vi "Choix des parametres.vi"() -> ()   [LabVIEW 2022 SP3]
uses:
  Enum/Enum 3.ctl
  Variables globales/Variable glob mails.vi
  Variables globales/Variable glob generale.vi
  Variables globales/Variable glob Leybold.vi
  Variables globales/Variable glob Edwards.vi
  Variables globales/Variable glob Keller.vi
  Variables globales/Variable glob Th.vi
  Variables globales/Variable glob Pt.vi
  Variables globales/Variables glob EUROTHERM.vi
  Variables globales/Variable globale compteurs.vi
  <vilib>/Utility/config.llb/NI_LVConfig.lvlib
panel:
  out "CUVE":string
  out "Refnum VI":refnum<vi>
  out "sortie d'erreur":errorcluster
  in  "Commande onglets 2":T1(tab)=enum."Temperatures Th"
  in  "Mails autres":string[](array[string]) caption="Mails autres (a renseigner) :"
  in  "Adresses mail IAS :":i32[](listbox)=[5] caption="Adresses mail IAS pour alertes :\n(selection par double clic)"
  in  "Commentaire dans le fichier :":string caption="Écrire éventuellement un commentaire qui sera inséré dans l'entête du fichier :"
  in  "Sous-dossier eventuel":string caption="Nom de l'expérience"
  in  "Nom manip":string caption="Nom de l'experience"
  in  "Sous-dossier precedents":u16(ring) items=["", "TEST_VADER_AVRIL2018"]
  in  "Experiences precedentes":u16(ring) items=["arretdu140716", "CAMERA FSI FM", "CAMERA FSI QM", "CAMERA HRI EUV FM", "CAMERA HRI EUV FM 2", "CAMERA HRI Lya FM", "essai blancdu070316", "FiltreFSI4et26du180716", "FiltreFSIFMmiroir3du50916", "FiltreFSIFmn6du010816", "FiltreFSIn30du270716", "FiltreFSIn32du210716", "FiltreFSIn5du250716", "FiltreFSIn6du290716", "FSI140416", "FSI150416", "FSIfiltreFMn13et25", "FSIfiltreFMn26", "FSIfiltreFMn4et26", "FSIfiltreQM180516", "HRIdu141015", "HRIdu151015", "HRIdu191015", "HRIdu271015", "Miroir2FSIdu30516", "NeptnXR90i", "NeptnXR90itest2", "POMPE RECEPTION", "PompNeptnxr40i", "PrepaNeptEUI", "Profils de température", "RGA", "test ablanc", "Test cDAQ", "Test programme", "TEST_VADER", "Testblanccam1et2du031215", "testmontage a blanc camdu270916", "tests camdu270916", "TESTS_LS340", "testsablanc", "testsBlancdu290916", "Testscam1et2du110216", "Testscam1et2du1mars16", "Testscam1et2du21mars16", "testscam1et2du300316", "testscamdu040416", "Testscaméra080216", "Testscaméra290116", "testscrycooleretbrides", "TestsEchandu281116", "échantHriFsi031016"]
  out "Chemin DATA local":path caption="Chemin DATA local :"
  in  "Chemin DATA distant":path caption="Chemin DATA distant :"
  in  "Chemin sauvegarde":path caption="Chemin sauvegarde :"
  out "Ports COM LEYBOLD":refnum<visa-resource-name>[](array[refnum])
  in  "Nom des jauges\nLEYBOLD":string[](array[string])
  in  "Selection\nLEYBOLD":bool[](array[boolean])
  out "Val LEYBOLD":string[](array[string]) caption="Valeurs\nLEYBOLD\ninstantanees"
  out "Val Grappes":string[](array[string]) caption="Valeurs Grappes\ninstantanees"
  in  "Selection\nGrappes":bool[](array[boolean])
  in  "Grappes":string[][](array[string])
  out "Ports COM EDWARDS":refnum<visa-resource-name>[](array[refnum])
  in  "Selection EDWARDS":bool[][](array[boolean])
  in  "Nom des jauges EDWARDS":string[][](array[string])
  out "Val EDWARDS":string[][](array[string]) caption="Valeurs EDWARDS instantanees"
  out "Nom de la tache Th associee":refnum<k21>
  in  "Tableau Th":T2(array[cluster])=[{"Test Th"=[], "Selection Th"=[TRUE, TRUE, FALSE, FALSE, TRUE, TRUE, FALSE, FALSE], "Tableau"=["Th1", "Th2", "Th3", "Th4", "Th5", "Th6", "Th7", "Th8"], "Noms Thermocouples :"=["SCXI1-Th1", "SCXI1-Th2", "SCXI1-Th3", "SCXI1-Th4", "SCXI1-Th5", "SCXI1-Th6", "SCXI1-Th7", "SCXI1-Th8"]}, {"Test Th"=[], "Selection Th"=[TRUE, TRUE, TRUE, TRUE, TRUE, TRUE, TRUE, TRUE], "Tableau"=["Th1", "Th2", "Th3", "Th4", "Th5", "Th6", "Th7", "Th8"], "Noms Thermocouples :"=["Thermocouple1", "Thermocouple2", "Thermocouple3", "Thermocouple4", "Thermocouple5", "Thermocouple6", "Thermocouple7", "Thermocouple8"]}]
  in  "Th n°":u8=1 caption="chassis n°" min=1
  in  "Tableau Pt":T3(array[cluster])=[{"Test Pt"=[], "Sélection Pt"=[TRUE, TRUE, FALSE, FALSE, TRUE, TRUE, FALSE, FALSE], "Tableau"=["Th1", "Th2", "Th3", "Th4", "Th5", "Th6", "Th7", "Th8"], "Noms Platines :"=["SCXI1-Th1", "SCXI1-Th2", "SCXI1-Th3", "SCXI1-Th4", "SCXI1-Th5", "SCXI1-Th6", "SCXI1-Th7", "SCXI1-Th8"]}, {"Test Pt"=[], "Sélection Pt"=[TRUE, TRUE, TRUE, TRUE, TRUE, TRUE, TRUE, TRUE], "Tableau"=["Th1", "Th2", "Th3", "Th4", "Th5", "Th6", "Th7", "Th8"], "Noms Platines :"=["Thermocouple1", "Thermocouple2", "Thermocouple3", "Thermocouple4", "Thermocouple5", "Thermocouple6", "Thermocouple7", "Thermocouple8"]}]
  in  "Pt n°":u8=1 caption="chassis n°" min=1
  out "Nom de la tache Pt associee":refnum<k21>
  out "Donnees reg":T4(array[cluster])
  in  "Reg dispo":T5(array[cluster])
  in  "Port COM REG":u16(ring) items=["COM6"]
  out "Adresses des jauges":i16[](array[numeric])
  out "Port COM KELLER (RS485)":refnum<visa-resource-name>
  out "Val KELLER":string[](array[string]) caption="Valeurs\nKELLER\ninstantanees"
  in  "Selection\nKELLER":bool[](array[boolean])
  in  "Nom des jauges KELLER":string[](array[string])
  in  "Temps pour débit":u16=3601 caption="Intervale de temps (s) pour debit" min=1
  out "data compteurs":string[](array[string])
  in  "Init compteurs (m3)":dbl[](array[numeric]) format="%.2f"
  in  "Selection":bool[](array[boolean])
  out "Noms des compteurs":string[](array[string])
  out "Nom de la tâche compteurs":refnum<k21>
  in  "annuler":bool
  in  "stop":bool
  # "choix des parametres"
  # "Ce logiciel et les informations qu'il contient, sont la propriété de l’IAS et ne peuvent être diffusés sans l’autorisation de la Station d’étalonnage"
  # "LES VALEURS AFFICHEES DANS LES TABLEAUX \"TEST\" CORRESPONDENT A UNE ACQUISITION TOUTES LES\nSECONDES SANS ENREGISTREMENT\n\nSEULES LES VOIES SÉLECTIONNEES SERONT ENSUITE ENREGISTREES"
  # "Définition du nom du dossier d'enregistrement des données.\nChoisir dans la liste de gauche ou écrire un nouveau nom dans la case de droite.\n\nLes fichiers seront écrits dans : D:\\Data\\CUVE\\Expérience\\(Sous-dossier\\)Année\\mois"
  # "Sélectionner les thermocouples"
  # "Sélectionner les platines du cDAQ"
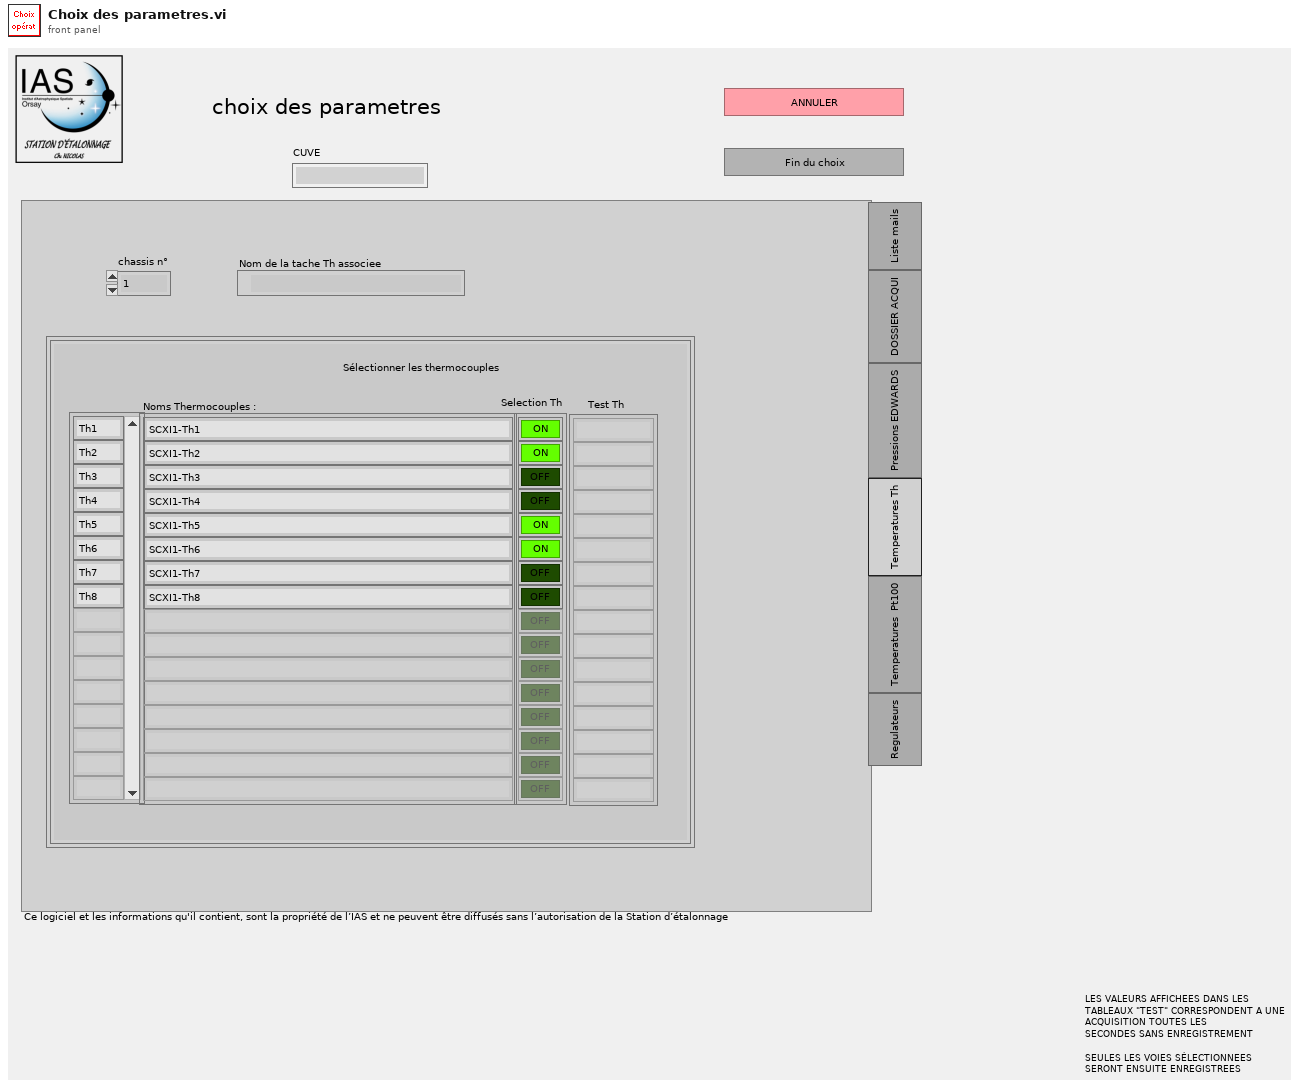
[diagram p1: front panel]
types:
  T1 = enum32{"Liste mails", "DOSSIER ACQUI", "Pressions LEYBOLD", "Pressions EDWARDS", "Temperatures Th", "Temperatures  Pt100", "Regulateurs", "Pressions KELLER", "Compteurs"}
  T2 = cluster{"Test Th":string[], "Selection Th":bool[], "Tableau":string[], "Noms Thermocouples :":string[]}[]
  T3 = cluster{"Test Pt":string[], "Sélection Pt":bool[], "Tableau":string[], "Noms Platines :":string[]}[]
  T4 = cluster{"Données  1 COM":cluster{"Pt100 Mesure":string, "Pt100 Securite":string}[]}[]
  T5 = cluster{"1 COM reg":cluster{"Nom":string, "Adresse":u8, "sélect":bool}[]}[]
  T6 = typedef "Enum 3.ctl" = enum16{"init", "init mail", "acquisition en cours ?", "onglets visibles", "init pressions", "initTh", "init Pt", "init reg", "init compteurs", "init dossiers", "lancement acqui tout", "choix operateur", "arret acquisitions", "enregistrement var glob pres", "enregistrement var glob temp", "enregistrement var glob reg", "enregistrement var glob compt et dossiers", "creation dossiers", "enregistrement fichier config", "fin"}
  T7 = cluster{"Données  1 COM":cluster{"Pt100 Mesure":string, "Pt100 Sécurité":string}[]}[]
  T8 = cluster{"Nom":string, "Adresse":u8, "sélect":bool}[]
  T9 = cluster{"Pt Mesure":string, "Pt Sécurité":string}
  T10 = enum32{"Invalid", "Standard", "Closed", "Hidden", "Minimized", "Maximized"}
  T11 = typedef "LVPositionTypeDef.ctl" = cluster{"Left":i32, "Top":i32}
  T12 = typedef "LVBoundsTypeDef.ctl" = cluster{"Width":u32, "Height":u32}
  T13 = cluster{"Nom tache Th":refnum<k21>, "Noms des Th":string[], "Nb Th":i16, "Selection Th":bool[], "Nom Th selectionnes":string[]}[]
  T14 = cluster{"Test Th":string[], "Selection Th":bool[], "Tableau":string[], "Noms Thermocouples :":string[]}
  T15 = cluster{"Nom tache Pt":refnum<k21>, "Noms des Pt":string[], "Nb Pt":i16, "Selection Pt":bool[], "Nom Pt selectionnees":string[]}[]
  T16 = cluster{"Test Pt":string[], "Sélection Pt":bool[], "Tableau":string[], "Noms Platines :":string[]}
  T17 = cluster{"1 COM reg":cluster{"Nom":string, "Adresse":u8, "sélect":bool}[]}
  T18 = cluster{"Nom":string, "Adresse":u8, "sélect":bool}
  T19 = cluster{"Nom tache compteurs":refnum<k21>, "Noms des compteurs":string[], "Selection":bool[], "Init compteurs":dbl[], "Noms compteurs selectionnes":string[]}
  T20 = cluster{cluster{"Pt Mesure":string, "Pt Sécurité":string}[]}
  T21 = cluster{"Nom tache Th":refnum<k21>, "Noms des Th":string[], "Nb Th":i16, "Selection Th":bool[], "Nom Th selectionnes":string[]}
  T22 = cluster{"Nom tache Pt":refnum<k21>, "Noms des Pt":string[], "Nb Pt":i16, "Selection Pt":bool[], "Nom Pt selectionnees":string[]}
  T23 = typedef "NI_LVConfig.lvlib/Config Data RefNum.ctl" = refnum<k1>
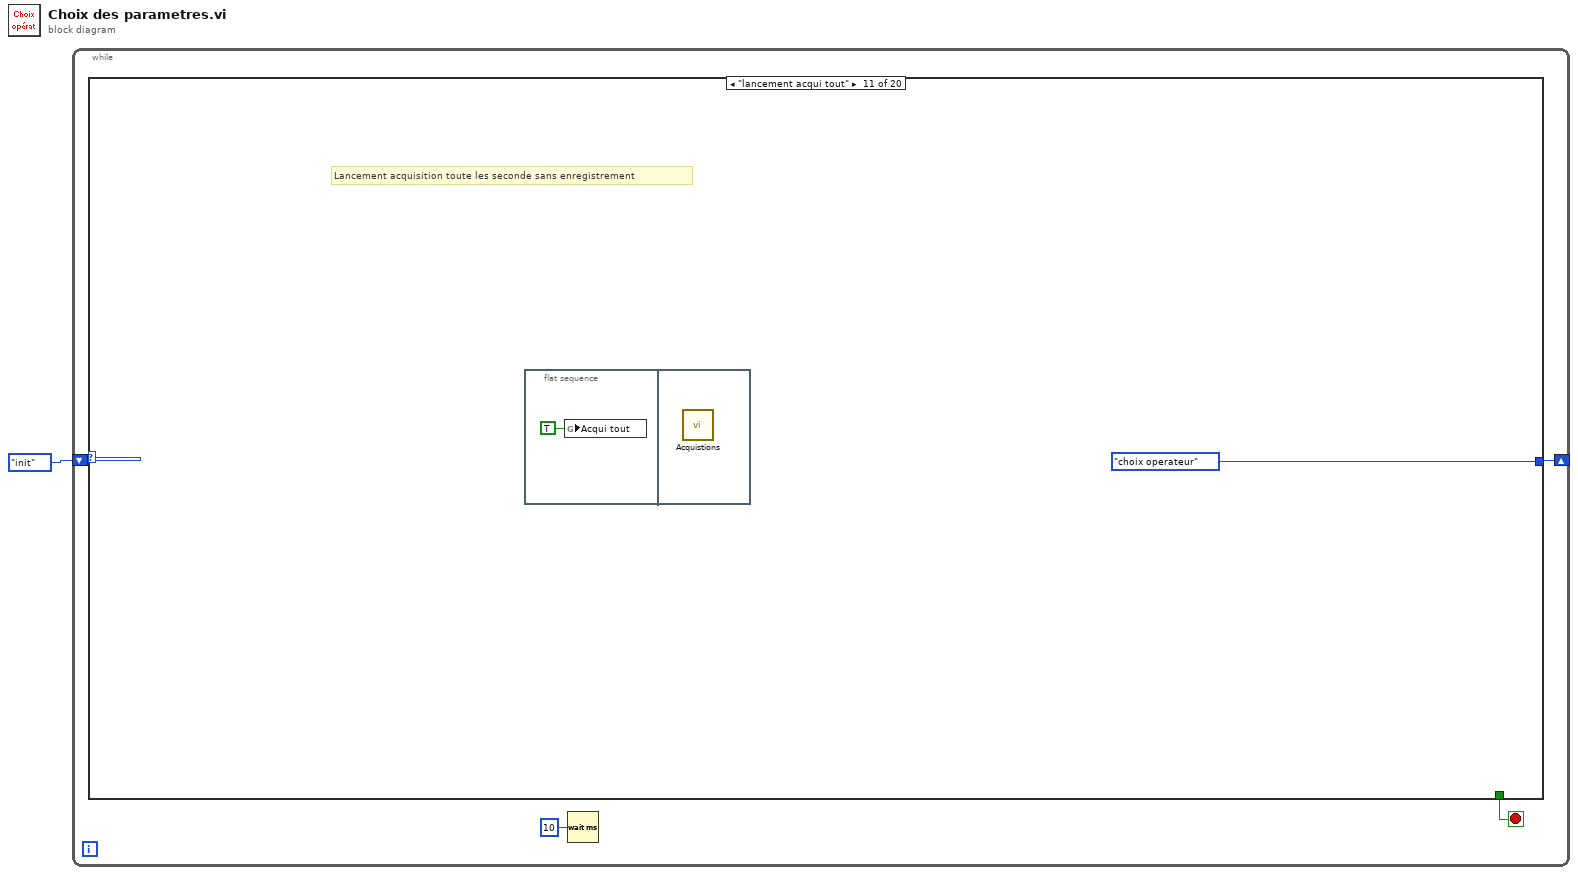
[diagram p0: block diagram]
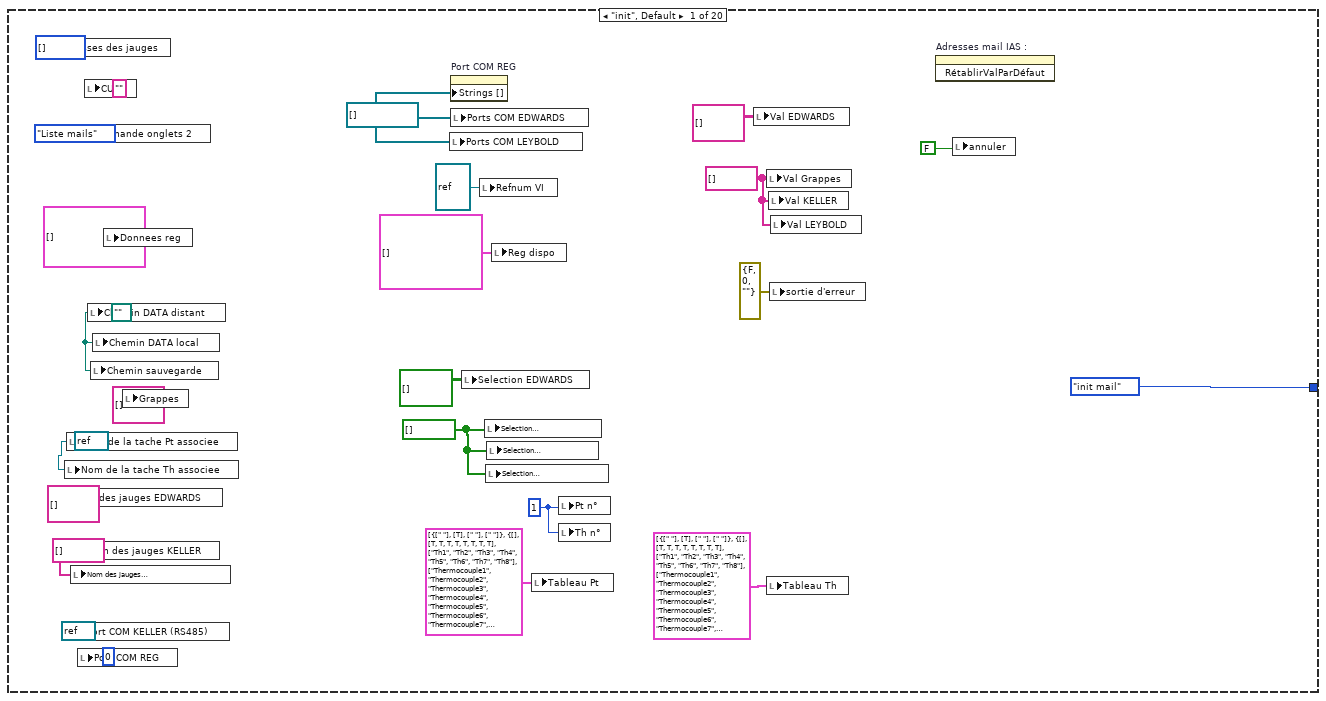
[diagram p2: hidden frame]
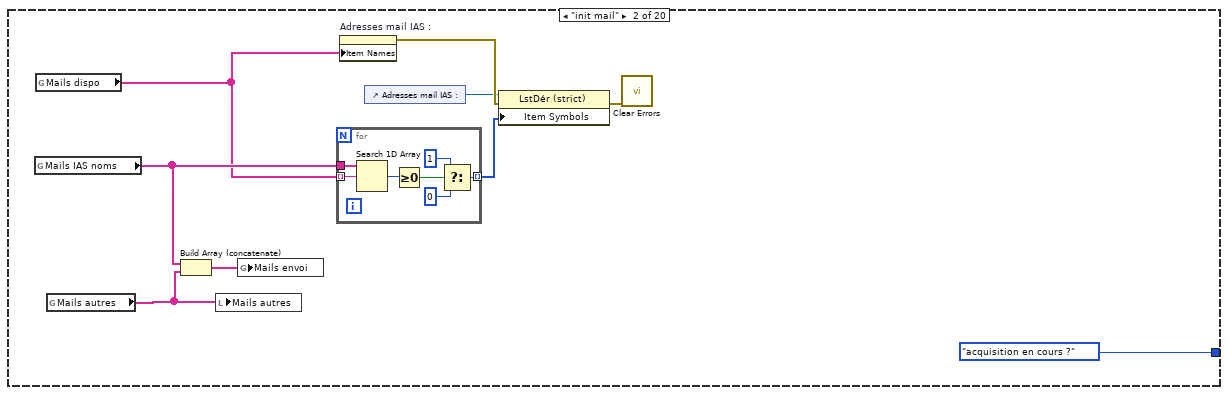
[diagram p3: hidden frame]
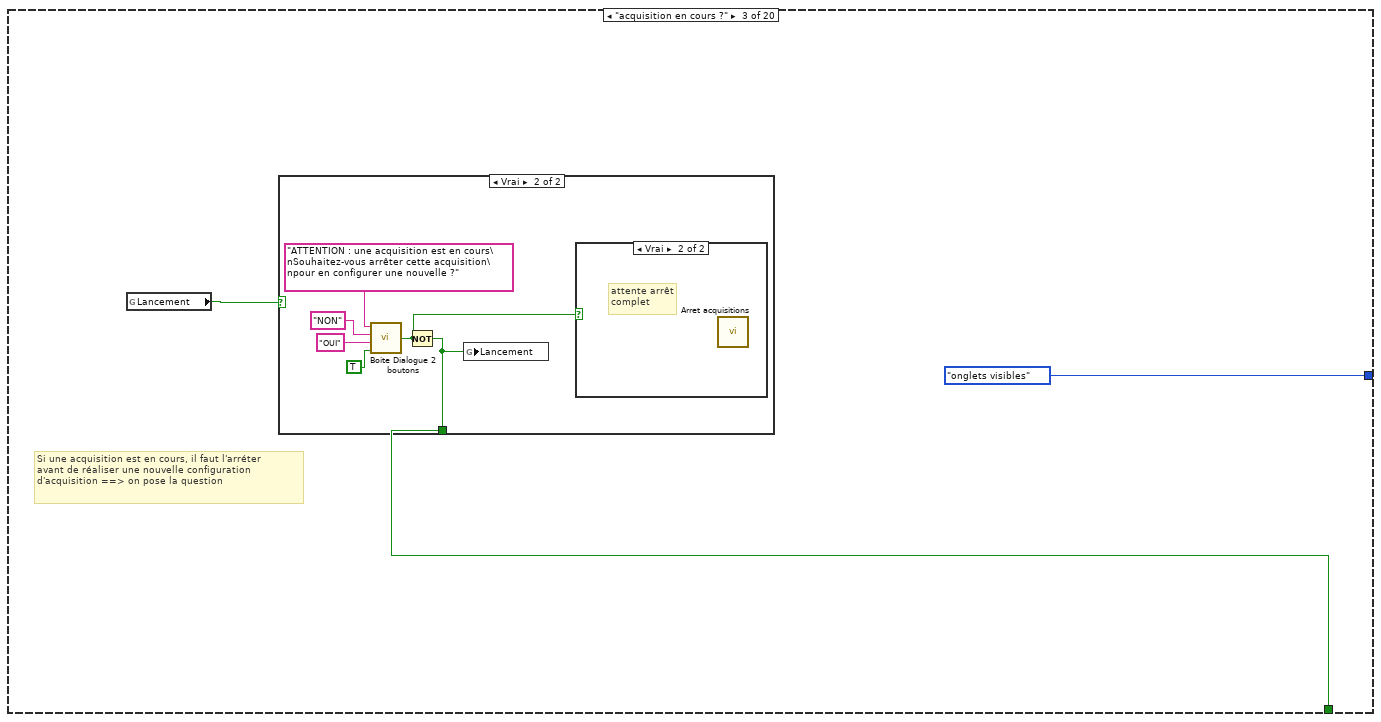
[diagram p4: hidden frame]
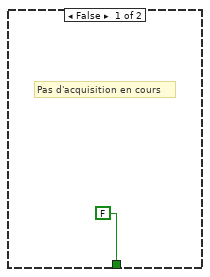
[diagram p5: hidden frame]
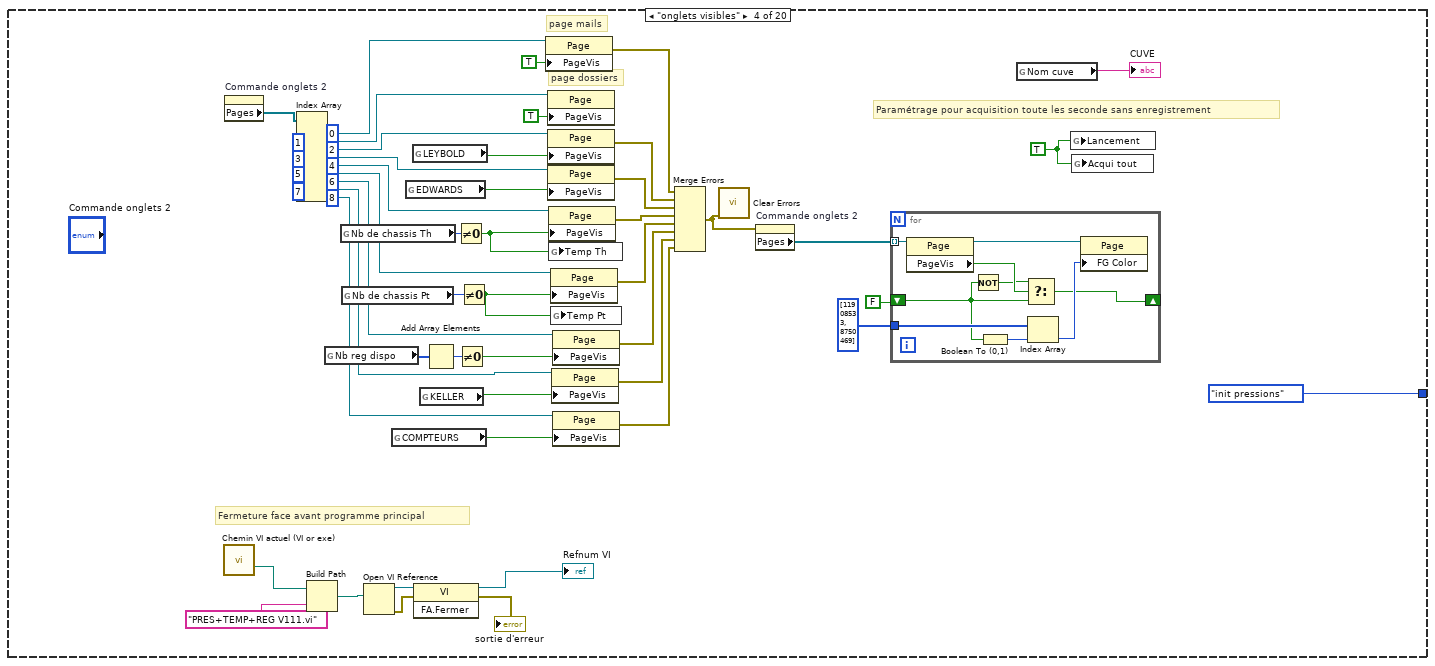
[diagram p7: hidden frame]
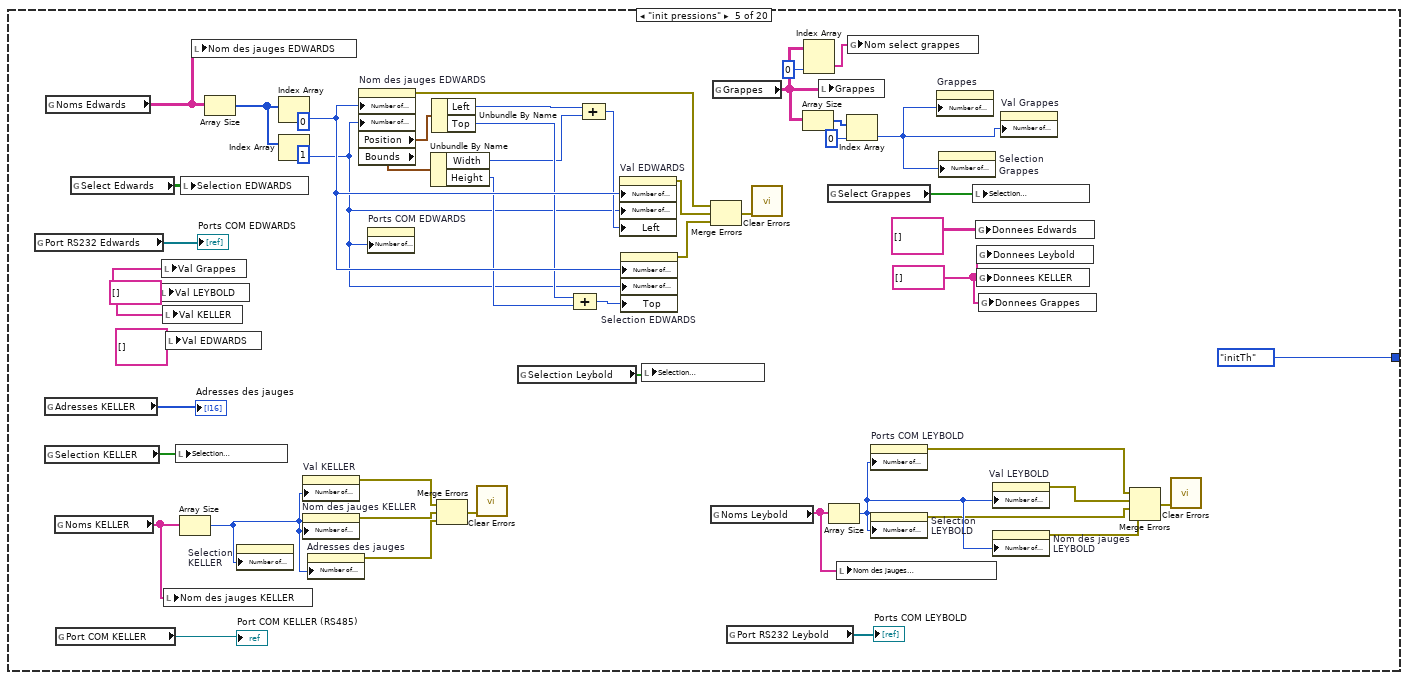
[diagram p8: hidden frame]
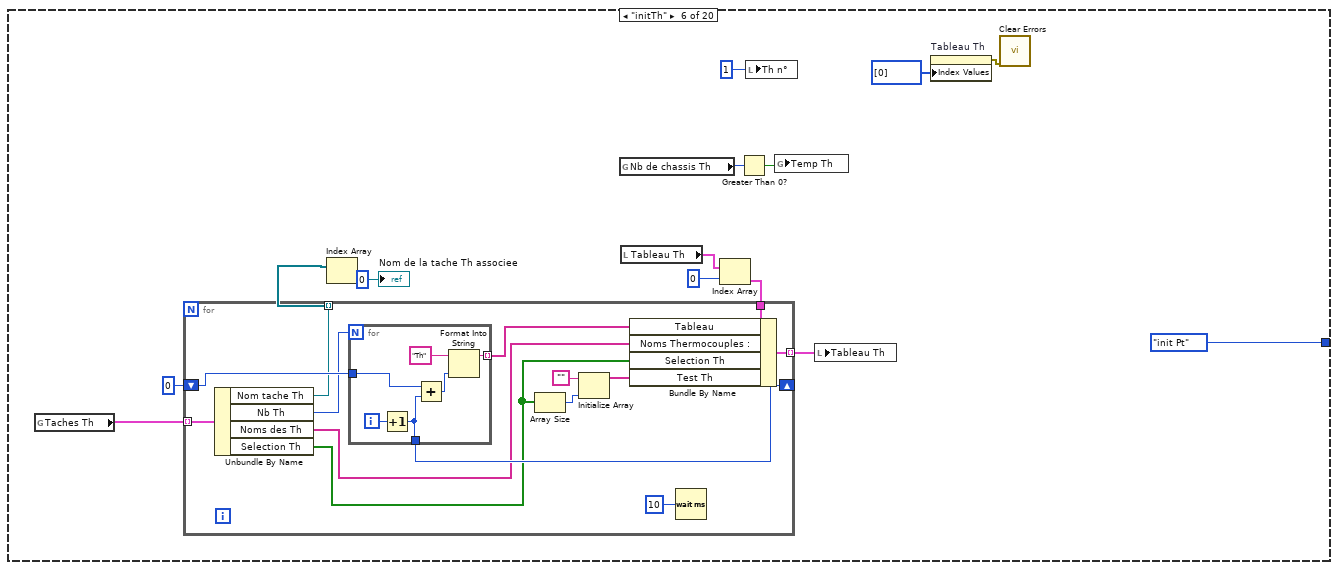
[diagram p9: hidden frame]
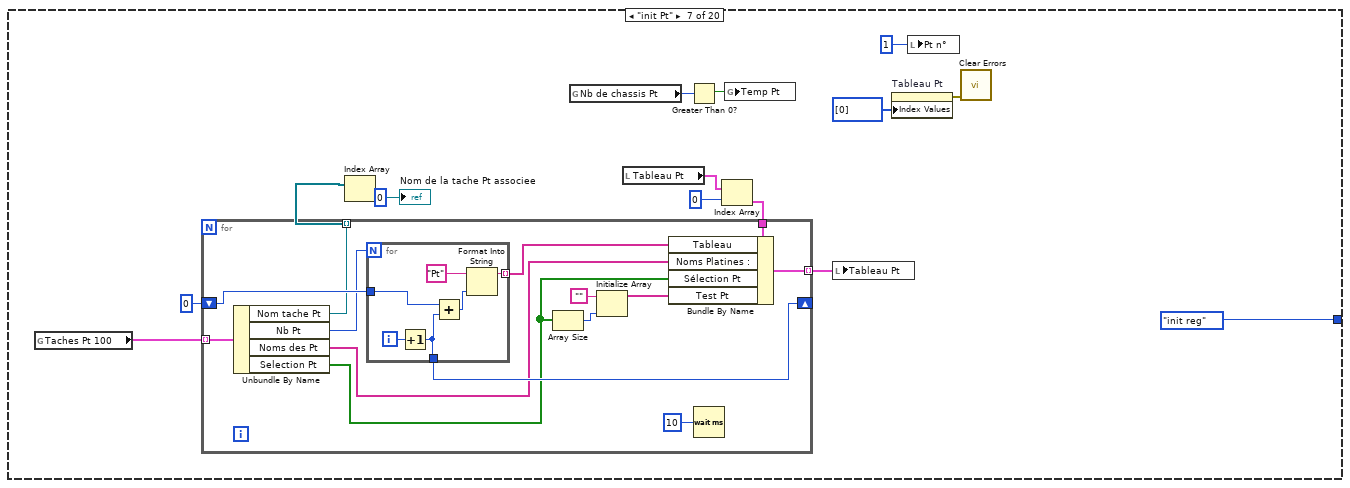
[diagram p10: hidden frame]
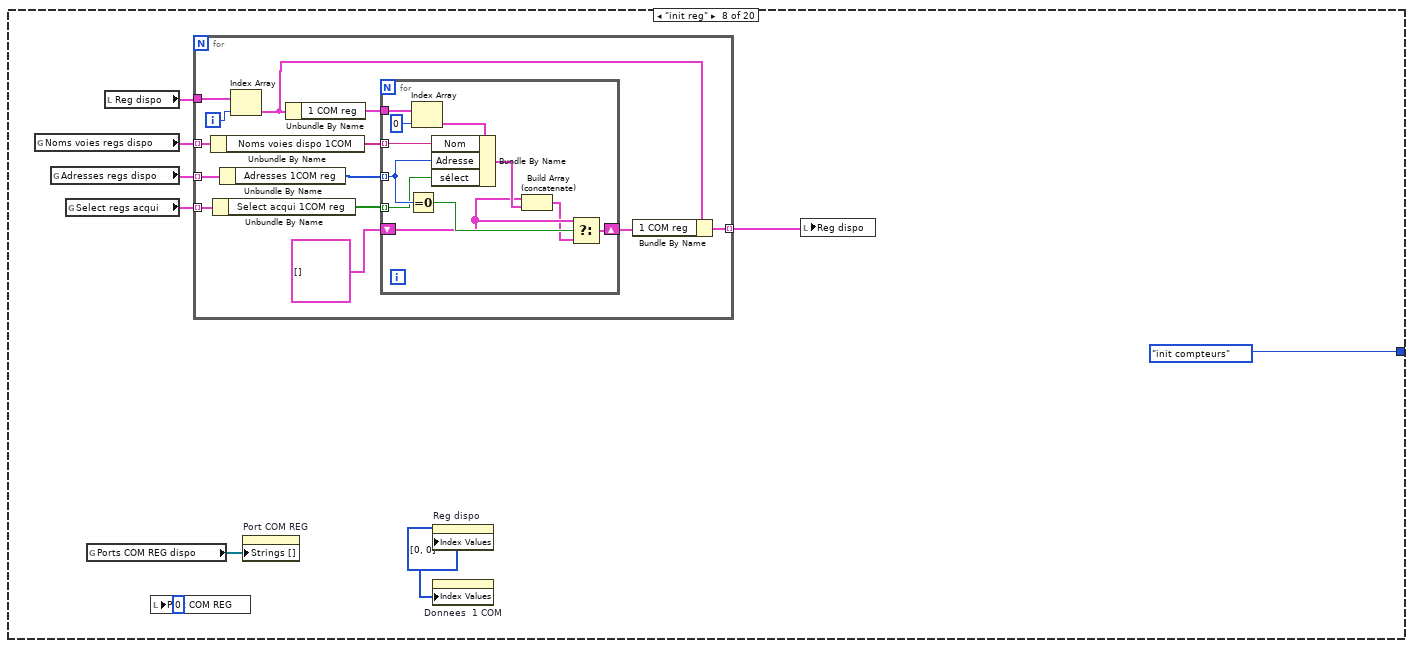
[diagram p11: hidden frame]
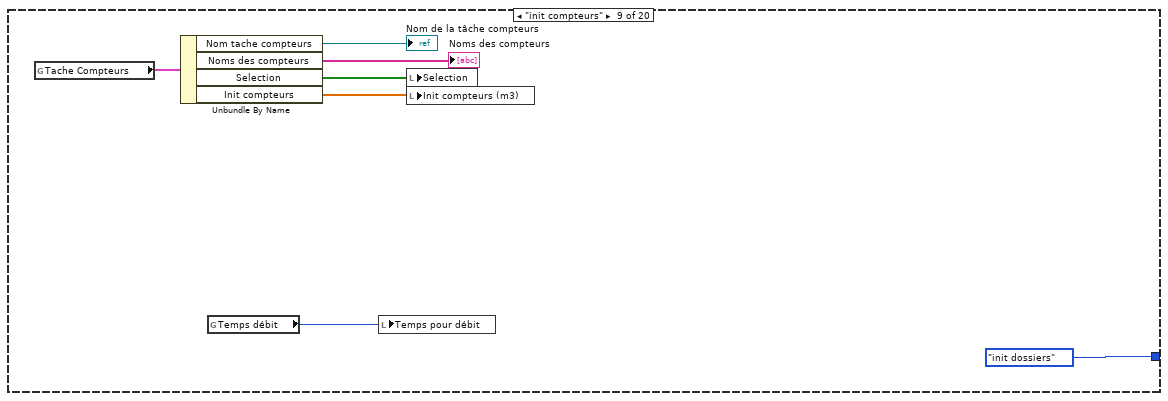
[diagram p12: hidden frame]
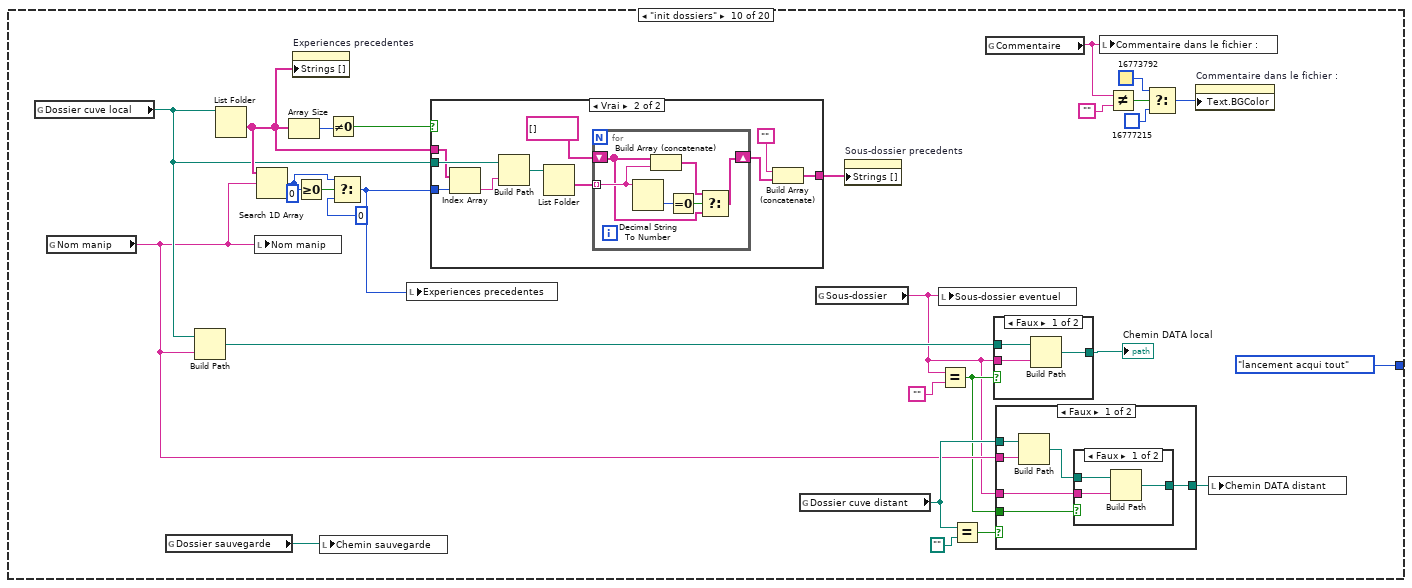
[diagram p13: hidden frame]
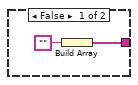
[diagram p17: hidden frame]
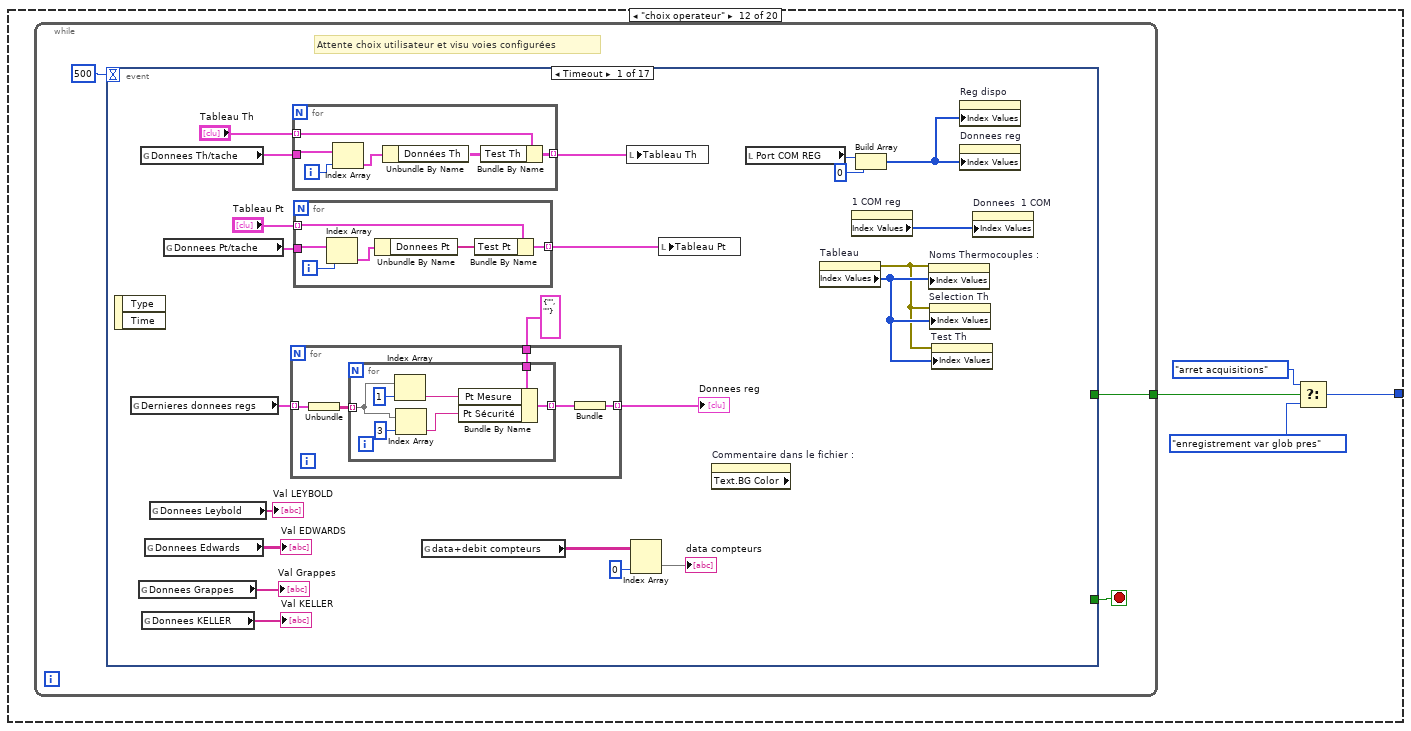
[diagram p18: hidden frame]
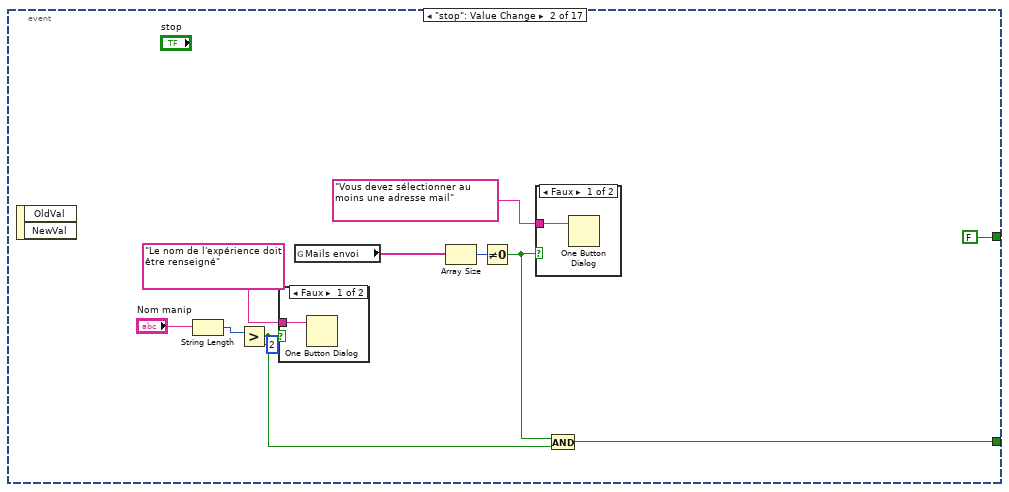
[diagram p19: hidden frame]
diagram:
  n1 = while {
    shift-right: [w4] -> _
    shift-left: Enum_3."init" ("Énum") -> [w5]
    stop <- w3 stop-if-true
    n2 = case shown="\"lancement acqui tout\"" w5 {
      tunnel: [Enum_3."init mail" ("Énum") Enum_3."acquisition en cours ?" ("Énum") Enum_3."onglets visibles" ("Énum") Enum_3."init pressions" ("Énum") Enum_3."initTh" ("Énum") Enum_3."init Pt" ("Énum") Enum_3."init reg" ("Énum") Enum_3."init compteurs" ("Énum") Enum_3."init dossiers" ("Énum") Enum_3."lancement acqui tout" ("Énum") Enum_3."choix operateur" ("Énum") w342 Enum_3."enregistrement var glob temp" ("Énum") Enum_3."enregistrement var glob reg" ("Énum") Enum_3."enregistrement var glob compt et dossiers" ("Énum") Enum_3."creation dossiers" ("Énum") Enum_3."enregistrement fichier config" ("Énum") Enum_3."arret acquisitions" ("Énum") Enum_3."fin" ("Énum") Enum_3."acquisition en cours ?" ("Énum")] -> w4
      tunnel: [_ _ w47 _ _ _ _ _ _ _ _ _ _ _ _ _ _ _ _ TRUE] -> w3
      frame "init", Default {
        w16 = string[] [] ("Val Grappes")
        w19 = bool[] [] ("Sélection\nGrappes")
        w10 = refnum<visa-resource-name>[] [] ("Ports COM EDWARDS")
        w23 = string[] [] ("Nom des jauges KELLER")
        w22 = refnum<k21> refnum ("Nom de la tâche Pt associée")
        w26 = path "" ("Dossier DATA distant")
        w18 = u8 1 ("Pt n°")
        n3 = local write "Adresses des jauges"(i16[] [] ("Adresses des jauges")) -> ()
        n4 = local write "Nom des jauges EDWARDS"(string[][] [] ("Nom des jauges EDWARDS")) -> ()
        n5 = local write "Nom de la tache Th associee"(w22) -> ()
        n6 = local write "Nom de la tache Pt associee"(w22) -> ()
        n7 = local write "Nom des jauges KELLER"(w23) -> ()
        n8 = local write "Nom des jauges\nLEYBOLD"(w23) -> ()
        n9 = local write "Port COM KELLER (RS485)"(refnum<visa-resource-name> refnum ("Port COM JUMO (RS485)")) -> ()
        n10 = local write "Commande onglets 2"(T1."Liste mails" ("Commande onglets 2")) -> ()
        n11 = local write "Port COM REG"(u16 0) -> ()
        n12 = local write "CUVE"("" ("CUVE")) -> ()
        n13 = local write "Chemin DATA distant"(w26) -> ()
        n14 = local write "Chemin sauvegarde"(w26) -> ()
        n15 = local write "Chemin DATA local"(w26) -> ()
        n16 = local write "Donnees reg"(T7 [] ("Donnees reg")) -> ()
        n17 = local write "Grappes"(string[][] [] ("Grappes")) -> ()
        n18 = local write "Ports COM LEYBOLD"(w10) -> ()
        n19 = property on="Port COM REG" class="MDér (strict)"("Strings []"=w10) -> ()  [unwired: 2 in, 2 out]
        n20 = local write "Ports COM EDWARDS"(w10) -> ()
        n21 = local write "Selection EDWARDS"(bool[][] [] ("Sélection EDWARDS")) -> ()
        n22 = local write "Refnum VI"(refnum<vi> refnum ("Refnum VI")) -> ()
        n23 = local write "Selection\nGrappes"(w19) -> ()
        n24 = local write "Selection\nLEYBOLD"(w19) -> ()
        n25 = local write "Selection\nKELLER"(w19) -> ()
        n26 = local write "Reg dispo"(T5 [] ("Reg dispo")) -> ()
        n27 = local write "Tableau Pt"(T3 [{"Test Pt"=[" "], "Sélection Pt"=[TRUE], "Tableau"=[" "], "Noms Platines :"=[" "]}, {"Test Pt"=[], "Sélection Pt"=[TRUE, TRUE, TRUE, TRUE, TRUE, TRUE, TRUE, TRUE], "Tableau"=["Th1", "Th2", "Th3", "Th4", "Th5", "Th6", "Th7", "Th8"], "Noms Platines :"=["Thermocouple1", "Thermocouple2", "Thermocouple3", "Thermocouple4", "Thermocouple5", "Thermocouple6", "Thermocouple7", "Thermocouple8"]}] ("Tableau Pt")) -> ()
        n28 = local write "Pt n°"(w18) -> ()
        n29 = local write "Th n°"(w18) -> ()
        n30 = local write "Val EDWARDS"(string[][] [] ("Val EDWARDS")) -> ()
        n31 = local write "Val Grappes"(w16) -> ()
        n32 = local write "Tableau Th"(T3 [{"Test Pt"=[" "], "Sélection Pt"=[TRUE], "Tableau"=[" "], "Noms Platines :"=[" "]}, {"Test Pt"=[], "Sélection Pt"=[TRUE, TRUE, TRUE, TRUE, TRUE, TRUE, TRUE, TRUE], "Tableau"=["Th1", "Th2", "Th3", "Th4", "Th5", "Th6", "Th7", "Th8"], "Noms Platines :"=["Thermocouple1", "Thermocouple2", "Thermocouple3", "Thermocouple4", "Thermocouple5", "Thermocouple6", "Thermocouple7", "Thermocouple8"]}] ("Tableau Pt")) -> ()
        n33 = local write "Val KELLER"(w16) -> ()
        n34 = local write "sortie d'erreur"(errorcluster {"status"=FALSE, "code"=0, "source"=""} ("sortie d'erreur")) -> ()
        n35 = local write "Val LEYBOLD"(w16) -> ()
        n36 = invoke on="Adresses mail IAS :" class="LstDér (strict)" method="RétablirValParDéfaut"() -> ()  [unwired: 3 in, 3 out]
        n37 = local write "annuler"(FALSE) -> ()
      }
      frame "init mail" {
        n38 = global read "Variable glob mails.vi" "Mails IAS noms"() -> (w33:string[])
        n39 = global read "Variable glob mails.vi" "Mails dispo"() -> (w30:string[])
        n40 = global read "Variable glob mails.vi" "Mails autres"() -> (w32:string[])
        n41 = Build Array (concatenate)(w33, w32) -> (w31:string[])
        n42 = local write "Mails autres"(w32) -> ()
        n43 = global write "Variable glob mails.vi" "Mails envoi"(w31) -> ()
        n44 = for {
          tunnel: w33 -> [w45]
          tunnel: w30 -> [w44] mode=indexing
          tunnel: [w39] -> w35 mode=indexing
          n45 = Search 1D Array(1D array=w45, element=w44) -> (index of element=w43:i32)  [unwired: 1 in]
          n46 = Greater Or Equal To 0?(x=w43) -> (x >= 0?=w42:bool)
          n47 = Select(t=1 ("cas vrai"), s=w42, f=0) -> (s? t:f=w39:i32)
        }
        n48 = property on="Adresses mail IAS :" class="LstDér (strict)"("Item Names"=w30) -> (error out=w36:errorcluster)  [unwired: 2 in, 1 out]
        n49 = control-ref of="Adresses mail IAS :"() -> (w34:refnum<vi>)
        n50 = property class="LstDér (strict)"(reference=w34, error in=w36, "Item Symbols"=w35) -> (error out=w37:errorcluster)  [unwired: 1 out]
        n51 = call <vilib>:"Clear Errors.vi"("error in (no error)"=w37) -> ()  [unwired: 5 in, 2 out]
      }
      frame "acquisition en cours ?" {
        # "Si une acquisition est en cours, il faut l'arréter\navant de réaliser une nouvelle configuration\nd'acquisition ==> on pose la question"
        n52 = global read "Variable glob generale.vi" "Lancement"() -> (w48:bool)
        n53 = case shown="Vrai" w48 {
          tunnel: [FALSE w55] -> w47
          frame False {
            # "Pas d'acquisition en cours"
          }
          frame True {
            n54 = call "Boite Dialogue 2 boutons.vi"("bouton droit visible ?"=TRUE, "Texte bouton droit"="OUI" ("Nom du bouton V (\"OK\")"), "Texte bouton gauche"="NON" ("Nom du bouton F (\"Annuler\")"), "Message"="ATTENTION : une acquisition est en cours\nSouhaitez-vous arrêter cette acquisition\npour en configurer une nouvelle ?" ("message")) -> ("Bouton droit ?"=w51:bool)
            n55 = Not(x=w51) -> (.not. x?=w55:bool)
            n56 = global write "Variable glob generale.vi" "Lancement"(w55) -> ()
            n57 = case shown="Vrai" w51 {
              frame False {
              }
              frame True {
                # "attente arrêt\ncomplet"
                n58 = call "Arret acquisitions.vi"() -> ()  [unwired: 12 in]
              }
            }
          }
        }
      }
      frame "onglets visibles" {
        w99 = TRUE
        # "page dossiers"
        # "page mails"
        # "Paramétrage pour acquisition toute les seconde sans enregistrement"
        # "Fermeture face avant programme principal"
        n59 = call "Chemin VI actuel (VI or exe).vi"() -> ("VI or executable installation directory"=w83:path)  [unwired: 14 in, 1 out]
        n60 = property on="Commande onglets 2" class="Onglet (strict)"() -> ("Pages"=w109:refnum<vi>[])  [unwired: 2 in, 2 out]
        n61 = Index Array(array=w109, index #1=0 ("indice"), index #2=1 ("indice"), index #3=2 ("indice"), index #4=3 ("indice"), index #5=4 ("indice"), index #6=5 ("indice"), index #7=6 ("indice"), index #8=7 ("indice"), index #9=8 ("indice")) -> (element #1=w79:refnum<vi>, element #2=w64:refnum<vi>, element #3=w63:refnum<vi>, element #4=w62:refnum<vi>, element #5=w61:refnum<vi>, element #6=w60:refnum<vi>, element #7=w59:refnum<vi>, element #8=w58:refnum<vi>, element #9=w56:refnum<vi>)
        n62 = Build Path(base path=w83, name or relative path="PRES+TEMP+REG V111.vi" ("nom ou chemin relatif")) -> (appended path=w95:path)
        n63 = global read "Variables glob EUROTHERM.vi" "Nb reg dispo"() -> (w81:u8[])
        n64 = global read "Variable glob Th.vi" "Nb de chassis Th"() -> (w107:u8)
        n65 = global read "Variable glob Pt.vi" "Nb de chassis Pt"() -> (w108:u8)
        n66 = Open VI Reference(vi path=w95) -> (vi reference=w93:refnum<vi>, error out=w92:errorcluster)  [unwired: 5 in]
        n67 = global read "Variable globale compteurs.vi" "COMPTEURS"() -> (w71:bool)
        n68 = global read "Variable glob Edwards.vi" "EDWARDS"() -> (w106:bool)
        n69 = global read "Variable glob Leybold.vi" "LEYBOLD"() -> (w105:bool)
        n70 = invoke class="VI" method="FA.Fermer"(reference=w93, error in=w92) -> (reference out=→"Refnum VI":refnum<vi>, error out=→"sortie d'erreur":errorcluster)  [unwired: 1 in, 1 out]
        n71 = global read "Variable glob Keller.vi" "KELLER"() -> (w66:bool)
        n72 = Add Array Elements(numeric array=w81) -> (sum=w80:u8)
        n73 = Not Equal To 0?(x=w107) -> (x != 0?=w69:bool)
        n74 = Not Equal To 0?(x=w80) -> (x != 0?=w67:bool)
        n75 = Not Equal To 0?(x=w108) -> (x != 0?=w68:bool)
        n76 = property class="Page"(reference=w79, "PageVis"=TRUE ("Page visible")) -> (error out=w77:errorcluster)  [unwired: 1 in, 1 out]
        n77 = property class="Page"(reference=w64, "PageVis"=TRUE ("Page visible")) -> ()  [unwired: 1 in, 2 out]
        n78 = property class="Page"(reference=w63, "PageVis"=w105) -> (error out=w91:errorcluster)  [unwired: 1 in, 1 out]
        n79 = property class="Page"(reference=w62, "PageVis"=w106) -> (error out=w88:errorcluster)  [unwired: 1 in, 1 out]
        n80 = property class="Page"(reference=w61, "PageVis"=w69) -> (error out=w87:errorcluster)  [unwired: 1 in, 1 out]
        n81 = global write "Variable glob Th.vi" "Temp Th"(w69) -> ()
        n82 = property class="Page"(reference=w60, "PageVis"=w68) -> (error out=w89:errorcluster)  [unwired: 1 in, 1 out]
        n83 = global write "Variable glob Pt.vi" "Temp Pt"(w68) -> ()
        n84 = property class="Page"(reference=w58, "PageVis"=w66) -> (error out=w84:errorcluster)  [unwired: 1 in, 1 out]
        n85 = property class="Page"(reference=w59, "PageVis"=w67) -> (error out=w90:errorcluster)  [unwired: 1 in, 1 out]
        n86 = property class="Page"(reference=w56, "PageVis"=w71) -> (error out=w70:errorcluster)  [unwired: 1 in, 1 out]
        n87 = Merge Errors(w77, w91, w88, w87, w89, w90, w84, w70) -> (w74:errorcluster)
        n88 = call <vilib>:"Clear Errors.vi"("error in (no error)"=w74) -> ()  [unwired: 5 in, 2 out]
        n89 = property on="Commande onglets 2" class="Onglet (strict)"(error in=w74) -> ("Pages"=w76:refnum<vi>[])  [unwired: 1 in, 2 out]
        n90 = for {
          tunnel: w76 -> [w118] mode=indexing
          tunnel: u32[] [11908533, 8750469] ("Tableau") -> [w115]
          shift-right: [w110] -> _
          shift-left: FALSE -> [w111]
          n91 = property class="Page"(reference=w118) -> (reference out=w117:refnum<vi>, "PageVis"=w116:bool)  [unwired: 1 in, 1 out]
          n92 = Not(x=w111) -> (.not. x?=w112:bool)
          n93 = Boolean To (0,1)(Boolean=w111) -> (0, 1=w113:i16)
          n94 = Select(t=w112, s=w116, f=w111) -> (s? t:f=w110:bool)
          n95 = Index Array(array=w115, index=w113) -> (element=w114:u32)
          n96 = property class="Page"(reference=w117, "FG Color"=w114) -> ()  [unwired: 1 in, 2 out]
        }
        n97 = global read "Variable glob generale.vi" "Nom cuve"() -> (→"CUVE":string)
        n98 = global write "Variable glob generale.vi" "Lancement"(w99) -> ()
        n99 = global write "Variable glob generale.vi" "Acqui tout"(w99) -> ()
      }
      frame "init pressions" {
        w125 = string[] [] ("Données KELLER")
        w126 = string[] [] ("Valeurs\nLEYBOLD\ninstantanées")
        n100 = global read "Variable glob Edwards.vi" "Port RS232 Edwards"() -> (→"Ports COM EDWARDS":refnum<visa-resource-name>[])
        n101 = global read "Variable glob Keller.vi" "Adresses KELLER"() -> (→"Adresses des jauges":i16[])
        n102 = global read "Variable glob Keller.vi" "Selection KELLER"() -> (w168:bool[])
        n103 = global read "Variable glob Edwards.vi" "Noms Edwards"() -> (w153:string[][])
        n104 = global read "Variable glob Keller.vi" "Noms KELLER"() -> (w152:string[])
        n105 = global read "Variable glob Keller.vi" "Port COM KELLER"() -> (→"Port COM KELLER (RS485)":refnum<visa-resource-name>)
        n106 = global read "Variable glob Edwards.vi" "Select Edwards"() -> (w166:bool[][])
        n107 = local write "Val LEYBOLD"(w126) -> ()
        n108 = local write "Val Grappes"(w126) -> ()
        n109 = local write "Val KELLER"(w126) -> ()
        n110 = local write "Nom des jauges KELLER"(w152) -> ()
        n111 = local write "Val EDWARDS"(string[][] [] ("Valeurs EDWARDS instantanées")) -> ()
        n112 = local write "Selection\nKELLER"(w168) -> ()
        n113 = Array Size(array=w152) -> (size(s)=w144:i32)
        n114 = local write "Selection EDWARDS"(w166) -> ()
        n115 = local write "Nom des jauges EDWARDS"(w153) -> ()
        n116 = Array Size(array=w153) -> (size(s)=w154:i32[])
        n117 = property on="Selection\nKELLER" class="Tabl (strict)"("Number of Rows"=w144) -> ()  [unwired: 2 in, 2 out]
        n118 = Index Array(array=w154, index=0 ("indice")) -> (element=w165:i32)
        n119 = Index Array(array=w154, index=1 ("indice")) -> (element=w147:i32)
        n120 = property on="Val KELLER" class="Tabl (strict)"("Number of Rows"=w144) -> (error out=w136:errorcluster)  [unwired: 2 in, 1 out]
        n121 = property on="Nom des jauges KELLER" class="Tabl (strict)"("Number of Rows"=w144) -> (error out=w135:errorcluster)  [unwired: 2 in, 1 out]
        n122 = property on="Adresses des jauges" class="Tabl (strict)"("Number of Rows"=w144) -> (error out=w134:errorcluster)  [unwired: 2 in, 1 out]
        n123 = property on="Nom des jauges EDWARDS" class="Tabl (strict)"("Number of Rows"=w165, "Number of Columns"=w147) -> (error out=w140:errorcluster, "Position"=w158:T11, "Bounds"=w157:T12)  [unwired: 2 in, 1 out]
        n124 = property on="Ports COM EDWARDS" class="Tabl (strict)"("Number of Columns"=w147) -> ()  [unwired: 2 in, 2 out]
        n125 = Unbundle By Name(w157) -> ("Width"=w160:u32, "Height"=w162:u32)
        n126 = Unbundle By Name(w158) -> ("Left"=w159:i32, "Top"=w161:i32)
        n127 = Merge Errors(w136, w135, w134) -> (w133:errorcluster)
        n128 = call <vilib>:"Clear Errors.vi"("error in (no error)"=w133) -> ()  [unwired: 5 in, 2 out]
        n129 = global read "Variable glob Leybold.vi" "Selection Leybold"() -> (w167:bool[])
        n130 = Compound Arithmetic op=ADD(w161, w162) -> (w163:u32)
        n131 = Compound Arithmetic op=ADD(w159, w160) -> (w164:u32)
        n132 = property on="Val EDWARDS" class="Tabl (strict)"("Number of Rows"=w165, "Number of Columns"=w147, "Left"=w164) -> (error out=w138:errorcluster)  [unwired: 2 in, 1 out]
        n133 = property on="Selection EDWARDS" class="Tabl (strict)"("Number of Rows"=w165, "Number of Columns"=w147, "Top"=w163) -> (error out=w139:errorcluster)  [unwired: 2 in, 1 out]
        n134 = local write "Selection\nLEYBOLD"(w167) -> ()
        n135 = Merge Errors(w140, w138, w139) -> (w137:errorcluster)
        n136 = global read "Variable glob Leybold.vi" "Noms Leybold"() -> (w151:string[])
        n137 = global read "Variable glob Edwards.vi" "Grappes"() -> (w121:string[][])
        n138 = global read "Variable glob Leybold.vi" "Port RS232 Leybold"() -> (→"Ports COM LEYBOLD":refnum<visa-resource-name>[])
        n139 = call <vilib>:"Clear Errors.vi"("error in (no error)"=w137) -> ()  [unwired: 5 in, 2 out]
        n140 = Array Size(array=w121) -> (size(s)=w124:i32[])
        n141 = Index Array(array=w121, index (col)=0 ("indice désactivé (col)")) -> (element=w119:string[])  [unwired: 1 in]
        n142 = local write "Grappes"(w121) -> ()
        n143 = global read "Variable glob Edwards.vi" "Select Grappes"() -> (w127:bool[])
        n144 = Array Size(array=w151) -> (size(s)=w149:i32)
        n145 = local write "Nom des jauges\nLEYBOLD"(w151) -> ()
        n146 = Index Array(array=w124, index=0 ("indice")) -> (element=w122:i32)
        n147 = global write "Variable glob Edwards.vi" "Nom select grappes"(w119) -> ()
        n148 = property on="Ports COM LEYBOLD" class="Tabl (strict)"("Number of Rows"=w149) -> (error out=w131:errorcluster)  [unwired: 2 in, 1 out]
        n149 = property on="Selection\nLEYBOLD" class="Tabl (strict)"("Number of Rows"=w149) -> (error out=w129:errorcluster)  [unwired: 2 in, 1 out]
        n150 = property on="Grappes" class="Tabl (strict)"("Number of Rows"=w122) -> ()  [unwired: 2 in, 2 out]
        n151 = property on="Selection\nGrappes" class="Tabl (strict)"("Number of Rows"=w122) -> ()  [unwired: 2 in, 2 out]
        n152 = local write "Selection\nGrappes"(w127) -> ()
        n153 = global write "Variable glob Edwards.vi" "Donnees Edwards"(string[][] [] ("Données Edwards")) -> ()
        n154 = global write "Variable glob Leybold.vi" "Donnees Leybold"(w125) -> ()
        n155 = global write "Variable glob Keller.vi" "Donnees KELLER"(w125) -> ()
        n156 = global write "Variable glob Edwards.vi" "Donnees Grappes"(w125) -> ()
        n157 = property on="Val LEYBOLD" class="Tabl (strict)"("Number of Rows"=w149) -> (error out=w130:errorcluster)  [unwired: 2 in, 1 out]
        n158 = property on="Nom des jauges\nLEYBOLD" class="Tabl (strict)"("Number of Rows"=w149) -> (error out=w128:errorcluster)  [unwired: 2 in, 1 out]
        n159 = property on="Val Grappes" class="Tabl (strict)"("Number of Rows"=w122) -> ()  [unwired: 2 in, 2 out]
        n160 = Merge Errors(w131, w130, w129, w128) -> (w132:errorcluster)
        n161 = call <vilib>:"Clear Errors.vi"("error in (no error)"=w132) -> ()  [unwired: 5 in, 2 out]
      }
      frame "initTh" {
        n162 = global read "Variable glob Th.vi" "Taches Th"() -> (w169:T13)
        n163 = global read "Variable glob Th.vi" "Nb de chassis Th"() -> (w182:u8)
        n164 = local read "Tableau Th"() -> (w174:T2)
        n165 = Index Array(array=w174, index=0 ("indice")) -> (element=w173:T14)
        n166 = for {
          tunnel: [w197] -> w175 mode=indexing
          tunnel: w173 -> [w196]
          shift-right: [w191] -> _
          shift-left: 0 -> [w190]
          tunnel: w169 -> [w188] mode=indexing
          tunnel: [w186] -> w171 mode=indexing
          n167 = Unbundle By Name(w188) -> ("Nom tache Th"=w186:refnum<k21>, "Nb Th"=w187:i16, "Noms des Th"=w185:string[], "Selection Th"=w184:bool[])
          n168 = for {
            N: w187 -> [_]
            tunnel: [w200] -> w194 mode=indexing
            tunnel: [w199] -> w191
            tunnel: w190 -> [w198]
            i -> [w203]
            n169 = Increment(x=w203) -> (x+1=w199:i32)
            n170 = Add(x=w198, y=w199) -> (x+y=w202:i32)
            n171 = Format Into String(initial string="Th", w202) -> (resulting string=w200:string)  [unwired: 2 in, 1 out]
          }
          n172 = Array Size(array=w184) -> (size(s)=w189:i32)
          n173 = Initialize Array("", w189) -> (w192:string[])
          n174 = Bundle By Name(cluster=w196, "Tableau"=w194, "Noms Thermocouples :"=w185, "Selection Th"=w184, "Test Th"=w192) -> (w197:T14)
          n175 = Wait (ms)(milliseconds to wait=u32 10 ("attente (ms)")) -> ()  [unwired: 1 out]
        }
        n176 = Index Array(array=w171, index=0 ("indice")) -> (element=→"Nom de la tache Th associee":refnum<k21>)
        n177 = Greater Than 0?(x=w182) -> (x > 0?=w181:bool)
        n178 = local write "Th n°"(u8 1 ("SCXI n°")) -> ()
        n179 = global write "Variable glob Th.vi" "Temp Th"(w181) -> ()
        n180 = local write "Tableau Th"(w175) -> ()
        n181 = property on="Tableau Th" class="Tabl (strict)"("Index Values"=u32[] [0] ("Valeurs d'indice")) -> (error out=w178:errorcluster)  [unwired: 2 in, 1 out]
        n182 = call <vilib>:"Clear Errors.vi"("error in (no error)"=w178) -> ()  [unwired: 5 in, 2 out]
      }
      frame "init Pt" {
        n183 = global read "Variable glob Pt.vi" "Taches Pt 100"() -> (w205:T15)
        n184 = global read "Variable glob Pt.vi" "Nb de chassis Pt"() -> (w217:u8)
        n185 = local read "Tableau Pt"() -> (w208:T3)
        n186 = Greater Than 0?(x=w217) -> (x > 0?=w216:bool)
        n187 = Index Array(array=w208, index=0 ("indice")) -> (element=w207:T16)
        n188 = for {
          tunnel: [w232] -> w209 mode=indexing
          tunnel: w207 -> [w231]
          shift-right: [w226] -> _
          shift-left: 0 -> [w225]
          tunnel: w205 -> [w223] mode=indexing
          tunnel: [w221] -> w204 mode=indexing
          n189 = Unbundle By Name(w223) -> ("Nom tache Pt"=w221:refnum<k21>, "Nb Pt"=w222:i16, "Noms des Pt"=w220:string[], "Selection Pt"=w219:bool[])
          n190 = for {
            N: w222 -> [_]
            tunnel: [w235] -> w229 mode=indexing
            tunnel: [w234] -> w226
            tunnel: w225 -> [w233]
            i -> [w238]
            n191 = Increment(x=w238) -> (x+1=w234:i32)
            n192 = Add(x=w233, y=w234) -> (x+y=w237:i32)
            n193 = Format Into String(initial string="Pt", w237) -> (resulting string=w235:string)  [unwired: 2 in, 1 out]
          }
          n194 = Array Size(array=w219) -> (size(s)=w224:i32)
          n195 = Initialize Array("", w224) -> (w227:string[])
          n196 = Bundle By Name(cluster=w231, "Tableau"=w229, "Noms Platines :"=w220, "Sélection Pt"=w219, "Test Pt"=w227) -> (w232:T16)
          n197 = Wait (ms)(milliseconds to wait=u32 10 ("attente (ms)")) -> ()  [unwired: 1 out]
        }
        n198 = Index Array(array=w204, index=0 ("indice")) -> (element=→"Nom de la tache Pt associee":refnum<k21>)
        n199 = global write "Variable glob Pt.vi" "Temp Pt"(w216) -> ()
        n200 = local write "Tableau Pt"(w209) -> ()
        n201 = property on="Tableau Pt" class="Tabl (strict)"("Index Values"=u32[] [0] ("Valeurs d'indice")) -> (error out=w213:errorcluster)  [unwired: 2 in, 1 out]
        n202 = local write "Pt n°"(u8 1 ("n°")) -> ()
        n203 = call <vilib>:"Clear Errors.vi"("error in (no error)"=w213) -> ()  [unwired: 5 in, 2 out]
      }
      frame "init reg" {
        w239 = u32[] [0, 0] ("Valeurs d'indice")
        n204 = global read "Variables glob EUROTHERM.vi" "Noms voies regs dispo"() -> (w242:cluster{"Noms voies dispo 1COM":string[]}[])
        n205 = global read "Variables glob EUROTHERM.vi" "Adresses regs dispo"() -> (w240:cluster{"Adresses 1COM reg":u16[]}[])
        n206 = global read "Variables glob EUROTHERM.vi" "Select regs acqui"() -> (w241:cluster{"Select acqui 1COM reg":bool[]}[])
        n207 = global read "Variables glob EUROTHERM.vi" "Ports COM REG dispo"() -> (w246:refnum<visa-resource-name>[])
        n208 = local read "Reg dispo"() -> (w244:T5)
        n209 = local write "Port COM REG"(u16 0) -> ()
        n210 = for {
          tunnel: w242 -> [w253] mode=indexing
          tunnel: w240 -> [w251] mode=indexing
          tunnel: w244 -> [w258]
          tunnel: [w259] -> w243 mode=indexing
          tunnel: w241 -> [w249] mode=indexing
          i -> [w256]
          n211 = Unbundle By Name(w253) -> ("Noms voies dispo 1COM"=w252:string[])
          n212 = Unbundle By Name(w249) -> ("Select acqui 1COM reg"=w248:bool[])
          n213 = Unbundle By Name(w251) -> ("Adresses 1COM reg"=w250:u16[])
          n214 = Index Array(array=w258, index=w256) -> (element=w257:T17)
          n215 = Unbundle By Name(w257) -> ("1 COM reg"=w260:T8)
          n216 = for {
            tunnel: w260 -> [w270]
            tunnel: w252 -> [w271] mode=indexing
            tunnel: w250 -> [w266] mode=indexing
            shift-right: [w262] -> w255
            shift-left: T8 [] -> [w264]
            tunnel: w248 -> [w261] mode=indexing
            n217 = Equal To 0?(x=w266) -> (x = 0?=w265:bool)
            n218 = Index Array(array=w270, index=0 ("indice")) -> (element=w268:T18)
            n219 = Bundle By Name(cluster=w268, "Nom"=w271, "Adresse"=w266, "sélect"=w261) -> (w267:T18)
            n220 = Build Array (concatenate)(w264, w267) -> (w263:T8)
            n221 = Select(t=w264, s=w265, f=w263) -> (s? t:f=w262:T8)
          }
          n222 = Bundle By Name(cluster=w257, "1 COM reg"=w255) -> (w259:T17)
        }
        n223 = property on="Port COM REG" class="MDér (strict)"("Strings []"=w246) -> ()  [unwired: 2 in, 2 out]
        n224 = property on="Reg dispo" class="Tabl (strict)"("Index Values"=w239) -> ()  [unwired: 2 in, 2 out]
        n225 = property on="Donnees  1 COM" class="Tabl (strict)"("Index Values"=w239) -> ()  [unwired: 2 in, 2 out]
        n226 = local write "Reg dispo"(w243) -> ()
      }
      frame "init compteurs" {
        n227 = global read "Variable globale compteurs.vi" "Tache Compteurs"() -> (w277:T19)
        n228 = Unbundle By Name(w277) -> ("Nom tache compteurs"=→"Nom de la tâche compteurs":refnum<k21>, "Noms des compteurs"=→"Noms des compteurs":string[], "Selection"=w275:bool[], "Init compteurs"=w274:dbl[])
        n229 = global read "Variable globale compteurs.vi" "Temps débit"() -> (w272:u16)
        n230 = local write "Temps pour débit"(w272) -> ()
        n231 = local write "Selection"(w275) -> ()
        n232 = local write "Init compteurs (m3)"(w274) -> ()
      }
      frame "init dossiers" {
        n233 = global read "Variable glob generale.vi" "Dossier cuve local"() -> (w294:path)
        n234 = global read "Variable glob generale.vi" "Nom manip"() -> (w287:string)
        n235 = global read "Variable glob generale.vi" "Dossier sauvegarde"() -> (w295:path)
        n236 = Build Path(base path=w294, name or relative path=w287) -> (appended path=w293:path)
        n237 = List Folder(path=w294) -> (folder names=w305:string[])  [unwired: 3 in, 3 out]
        n238 = local write "Nom manip"(w287) -> ()
        n239 = Search 1D Array(1D array=w305, element=w287, start index (0)=0 ("indice de départ (0)")) -> (index of element=w298:i32)
        n240 = Array Size(array=w305) -> (size(s)=w303:i32)
        n241 = property on="Experiences precedentes" class="MDér (strict)"("Strings []"=w305) -> ()  [unwired: 2 in, 2 out]
        n242 = Greater Or Equal To 0?(x=w298) -> (x >= 0?=w299:bool)
        n243 = local write "Chemin sauvegarde"(w295) -> ()
        n244 = Not Equal To 0?(x=w303) -> (x != 0?=w304:bool)
        n245 = Select(t=w298, s=w299, f=u16 0) -> (s? t:f=w296:i32)
        n246 = local write "Experiences precedentes"(w296) -> ()
        n247 = case shown="Vrai" w304 {
          tunnel: w296 -> [_ w331]
          tunnel: w294 -> [_ w328]
          tunnel: [w322 w327] -> w301
          tunnel: w305 -> [_ w324]
          frame False {
            n248 = Build Array("") -> (w322:string[])
          }
          frame True {
            n249 = Index Array(array=w324, index=w331) -> (element=w329:string)
            n250 = Build Path(base path=w328, name or relative path=w329) -> (appended path=w330:path)
            n251 = List Folder(path=w330) -> (folder names=w333:string[])  [unwired: 3 in, 3 out]
            n252 = for {
              tunnel: w333 -> [w337] mode=indexing
              shift-right: [w335] -> w326
              shift-left: string[] [] -> [w334]
              n253 = Decimal String To Number(string=w337) -> (number=w339:i32)  [unwired: 2 in, 1 out]
              n254 = Build Array (concatenate)(w334, w337) -> (w336:string[])
              n255 = Equal To 0?(x=w339) -> (x = 0?=w338:bool)
              n256 = Select(t=w336, s=w338, f=w334) -> (s? t:f=w335:string[])
            }
            n257 = Build Array (concatenate)("", w326) -> (w327:string[])
          }
        }
        n258 = global read "Variable glob generale.vi" "Dossier cuve distant"() -> (w288:path)
        n259 = global read "Variable glob generale.vi" "Sous-dossier"() -> (w285:string)
        n260 = property on="Sous-dossier precedents" class="MDér (strict)"("Strings []"=w301) -> ()  [unwired: 2 in, 2 out]
        n261 = local write "Sous-dossier eventuel"(w285) -> ()
        n262 = Equal?(x=w285, y="") -> (x = y?=w286:bool)
        n263 = Equal?(x=w288, y=path "") -> (x = y?=w289:bool)
        n264 = global read "Variable glob generale.vi" "Commentaire"() -> (w279:string)
        n265 = case shown="Faux" w286 {
          tunnel: w293 -> [w320 w321]
          tunnel: w285 -> [w318 _]
          tunnel: [w319 w321] -> w292
          frame False {
            n266 = Build Path(base path=w320, name or relative path=w318) -> (appended path=w319:path)
          }
          frame True {
          }
        }
        "Chemin DATA local" <- w292
        n267 = case shown="Faux" w289 {
          tunnel: w288 -> [w311 w317]
          tunnel: [w307 w317] -> w284
          tunnel: w287 -> [w312 _]
          tunnel: w286 -> [w310 _]
          tunnel: w285 -> [w308 _]
          frame False {
            n268 = Build Path(base path=w311, name or relative path=w312) -> (appended path=w309:path)
            n269 = case shown="Faux" w310 {
              tunnel: w309 -> [w315 w316]
              tunnel: w308 -> [w313 _]
              tunnel: [w314 w316] -> w307
              frame False {
                n270 = Build Path(base path=w315, name or relative path=w313) -> (appended path=w314:path)
              }
              frame True {
              }
            }
          }
          frame True {
          }
        }
        n271 = local write "Commentaire dans le fichier :"(w279) -> ()
        n272 = Not Equal?(x=w279, y="") -> (x != y?=w281:bool)
        n273 = Select(t=u32 16773792, s=w281, f=u32 16777215) -> (s? t:f=w302:u32)
        n274 = property on="Commentaire dans le fichier :" class="Ch"("Text.BGColor"=w302) -> ()  [unwired: 2 in, 2 out]
        n275 = local write "Chemin DATA distant"(w284) -> ()
      }
      frame "lancement acqui tout" {
        # "Lancement acquisition toute les seconde sans enregistrement"
        n276 = flat-sequence {
          frame #0 {
            n277 = global write "Variable glob generale.vi" "Acqui tout"(TRUE ("Acqui tout")) -> ()
          }
          frame #1 {
            n278 = call "Acquistions.vi"() -> ()  [unwired: 4 in]
          }
        }
      }
      frame "choix operateur" {
        n279 = while {
          tunnel: [w346] -> w344
          stop <- w347 stop-if-true
          # "Attente choix utilisateur et visu voies configurées"
          n280 = event shown="[0] Timeout" {
            selector: _ -> [_ _ _ _ _ _ _ _ _ _ _ _ _ _ _ _ _]
            dyn-events: _ -> [_ _ _ _ _ _ _ _ _ _ _ _ _ _ _ _ _]
            timeout: u32 500 ("attente (ms)") -> [_ _ _ _ _ _ _ _ _ _ _ _ _ _ _ _ _]
            tunnel: [_ w397 TRUE _ _ _ _ _ _ _ _ _ _ _ _ _ _] -> w347
            tunnel: [_ FALSE TRUE _ _ _ _ _ _ _ _ _ _ _ _ _ _] -> w346
            event Timeout {
              n281 = event-data() -> ()  [unwired: 1 in, 2 out]
              n282 = global read "Variables glob EUROTHERM.vi" "Dernieres donnees regs"() -> (w358:cluster{"Dernieres donnees 1COM":string[][]}[])
              n283 = global read "Variable glob Edwards.vi" "Donnees Grappes"() -> (→"Val Grappes":string[])
              n284 = global read "Variable glob Th.vi" "Donnees Th/tache"() -> (w359:cluster{"Données Th":string[]}[])
              n285 = global read "Variable glob Keller.vi" "Donnees KELLER"() -> (→"Val KELLER":string[])
              n286 = global read "Variable glob Edwards.vi" "Donnees Edwards"() -> (→"Val EDWARDS":string[][])
              n287 = global read "Variable glob Leybold.vi" "Donnees Leybold"() -> (→"Val LEYBOLD":string[])
              n288 = global read "Variable glob Pt.vi" "Donnees Pt/tache"() -> (w368:cluster{"Donnees Pt":string[]}[])
              n289 = for {
                tunnel: [w371] -> w353 mode=indexing
                tunnel: T9 {"Pt Mesure"="", "Pt Sécurité"=""} ("Cluster") -> [w375]
                tunnel: w358 -> [w374] mode=indexing
                n290 = Unbundle(w374) -> ("Dernieres donnees 1COM"=w373:string[][])
                n291 = for {
                  tunnel: w373 -> [w380] mode=indexing
                  tunnel: [w377] -> w372 mode=indexing
                  tunnel: w375 -> [w376]
                  n292 = Index Array(array=w380, index=1 ("indice")) -> (element=w379:string)
                  n293 = Index Array(array=w380, index=3 ("indice")) -> (element=w378:string)
                  n294 = Bundle By Name(cluster=w376, "Pt Mesure"=w379, "Pt Sécurité"=w378) -> (w377:T9)
                }
                n295 = Bundle(w372) -> (w371:T20)  [unwired: 1 in]
              }
              "Donnees reg" <- w353
              n296 = for {
                tunnel: [w394] -> w370 mode=indexing
                tunnel: "Tableau Th" -> [w393] mode=indexing
                tunnel: w359 -> [w390]
                i -> [w391]
                n297 = Index Array(array=w390, index=w391) -> (element=w389:cluster{"Données Th":string[]})
                n298 = Unbundle By Name(w389) -> ("Données Th"=w392:string[])
                n299 = Bundle By Name(cluster=w393, "Test Th"=w392) -> (w394:T14)
              }
              n300 = for {
                tunnel: [w388] -> w367 mode=indexing
                tunnel: "Tableau Pt" -> [w387] mode=indexing
                tunnel: w368 -> [w384]
                i -> [w385]
                n301 = Index Array(array=w384, index=w385) -> (element=w383:cluster{"Donnees Pt":string[]})
                n302 = Unbundle By Name(w383) -> ("Donnees Pt"=w386:string[])
                n303 = Bundle By Name(cluster=w387, "Test Pt"=w386) -> (w388:T16)
              }
              n304 = global read "Variable globale compteurs.vi" "data+debit compteurs"() -> (w351:string[][])
              n305 = local write "Tableau Th"(w370) -> ()
              n306 = Index Array(array=w351, index (col)=0 ("indice désactivé (col)")) -> (element=→"data compteurs":string[])  [unwired: 1 in]
              n307 = local write "Tableau Pt"(w367) -> ()
              n308 = property on="Commentaire dans le fichier :" class="Ch" props=["Text", "BG Color"]() -> ()  [unwired: 2 in, 3 out]
              n309 = local read "Port COM REG"() -> (w356:u16)
              n310 = property on="Tableau" class="Tabl (strict)"() -> (error out=w364:errorcluster, "Index Values"=w365:u32[])  [unwired: 2 in, 1 out]
              n311 = property on="1 COM reg" class="Tabl (strict)"() -> ("Index Values"=w352:u32[])  [unwired: 2 in, 2 out]
              n312 = Build Array(w356, u16 0 ("élément")) -> (w354:u16[])
              n313 = property on="Noms Thermocouples :" class="Tabl (strict)"(error in=w364, "Index Values"=w365) -> ()  [unwired: 1 in, 2 out]
              n314 = property on="Selection Th" class="Tabl (strict)"(error in=w364, "Index Values"=w365) -> ()  [unwired: 1 in, 2 out]
              n315 = property on="Test Th" class="Tabl (strict)"(error in=w364, "Index Values"=w365) -> ()  [unwired: 1 in, 2 out]
              n316 = property on="Reg dispo" class="Tabl (strict)"("Index Values"=w354) -> ()  [unwired: 2 in, 2 out]
              n317 = property on="Donnees reg" class="Tabl (strict)"("Index Values"=w354) -> ()  [unwired: 2 in, 2 out]
              n318 = property on="Donnees  1 COM" class="Tabl (strict)"("Index Values"=w352) -> ()  [unwired: 2 in, 2 out]
            }
            event "stop": Value Change {
              n319 = event-data() -> ()  [unwired: 1 in, 2 out]
              n320 = String Length(string="Nom manip") -> (length=w403:i32)
              n321 = Greater?(x=w403, y=2) -> (0:w398:bool)
              n322 = case shown="Faux" w398 {
                tunnel: "Le nom de l'expérience doit être renseigné" -> [w406 _]
                frame False {
                  n323 = One Button Dialog(message=w406) -> ()  [unwired: 1 in, 1 out]
                }
                frame True {
                }
              }
              n324 = global read "Variable glob mails.vi" "Mails envoi"() -> (w395:string[])
              n325 = Array Size(array=w395) -> (size(s)=w405:i32)
              n326 = Not Equal To 0?(x=w405) -> (x != 0?=w399:bool)
              n327 = case shown="Faux" w399 {
                tunnel: "Vous devez sélectionner au moins une adresse mail" -> [w407 _]
                frame False {
                  n328 = One Button Dialog(message=w407) -> ()  [unwired: 1 in, 1 out]
                }
                frame True {
                }
              }
              n329 = And(x=w399, y=w398) -> (x .and. y?=w397:bool)
            }
            event "annuler": Value Change {
              n330 = event-data() -> ()  [unwired: 1 in, 2 out]
            }
            event "Adresses mail IAS :": Double Click {
              n331 = event-data() -> ("CtlRef"=w413:refnum<vi>)  [unwired: 1 in, 8 out]
              n332 = control-ref of="Adresses mail IAS :"() -> (w414:refnum<vi>)
              n333 = call "Mise a jour liste Selection.vi"("RéfCmde sélection"=w413, "Choisir capteur parmis"=w414) -> ("error out"=w415:errorcluster, "Capteurs choisit"=w410:string[])  [unwired: 8 in]
              n334 = call <vilib>:"Clear Errors.vi"("error in (no error)"=w415) -> ()  [unwired: 5 in, 2 out]
              n335 = global write "Variable glob mails.vi" "Mails IAS noms"(w410) -> ()
              n336 = global read "Variable glob mails.vi" "Mails autres"() -> (w411:string[])
              n337 = Build Array (concatenate)(w410, w411) -> (w412:string[])
              n338 = global write "Variable glob mails.vi" "Mails envoi"(w412) -> ()
            }
            event "Mails autres": Value Change {
              n339 = event-data() -> ("NewVal"=w418:string[])  [unwired: 1 in, 2 out]
              n340 = global read "Variable glob mails.vi" "Mails IAS noms"() -> (w416:string[])
              n341 = global write "Variable glob mails.vi" "Mails autres"(w418) -> ()
              n342 = Build Array (concatenate)(w416, w418) -> (w417:string[])
              n343 = global write "Variable glob mails.vi" "Mails envoi"(w417) -> ()
            }
            event "Selection EDWARDS": Value Change {
              n344 = event-data() -> ("NewVal"=w419:bool[][])  [unwired: 1 in, 4 out]
              n345 = for {
                tunnel: w419 -> [w421] mode=indexing
                i -> [w420]
                n346 = for {
                  tunnel: w421 -> [w424] mode=indexing
                  tunnel: w420 -> [w423]
                  i -> [w422]
                  n347 = case shown="Faux" w424 {
                    tunnel: w423 -> [w430 _]
                    tunnel: w422 -> [w429 _]
                    frame False {
                      n348 = local read "Nom des jauges EDWARDS"() -> (w431:string[][])
                      n349 = local read "Selection\nGrappes"() -> (w426:bool[])
                      n350 = Index Array(array=w431, index (row)=w430, index (col)=w429) -> (element=w427:string)
                      n351 = local read "Grappes"() -> (w428:string[][])
                      n352 = for {
                        tunnel: w428 -> [w438] mode=indexing
                        tunnel: w427 -> [w437]
                        tunnel: [w434] -> w425 mode=indexing
                        tunnel: w426 -> [w433] mode=indexing
                        n353 = Search 1D Array(1D array=w438, element=w437) -> (index of element=w436:i32)  [unwired: 1 in]
                        n354 = Greater Or Equal To 0?(x=w436) -> (x >= 0?=w435:bool)
                        n355 = Select(t=FALSE ("cas vrai"), s=w435, f=w433) -> (s? t:f=w434:bool)
                      }
                      n356 = local write "Selection\nGrappes"(w425) -> ()
                    }
                    frame True {
                    }
                  }
                }
              }
            }
            event "Selection\nGrappes": Value Change {
              n357 = event-data() -> ("NewVal"=w439:bool[])  [unwired: 1 in, 4 out]
              n358 = for {
                tunnel: w439 -> [w441] mode=indexing
                i -> [w440]
                n359 = case shown="Vrai" w441 {
                  tunnel: w440 -> [_ w443]
                  frame False {
                  }
                  frame True {
                    n360 = local read "Grappes"() -> (w444:string[][])
                    n361 = Index Array(array=w444, index (row)=w443) -> (element=w442:string[])  [unwired: 1 in]
                    n362 = for {
                      tunnel: w442 -> [w447] mode=indexing
                      n363 = local read "Nom des jauges EDWARDS"() -> (w448:string[][])
                      n364 = local read "Selection EDWARDS"() -> (w446:bool[][])
                      n365 = for {
                        tunnel: w448 -> [w456] mode=indexing
                        tunnel: w447 -> [w455]
                        tunnel: w446 -> [w450] mode=indexing
                        tunnel: [w449] -> w445 mode=indexing
                        n366 = Search 1D Array(1D array=w456, element=w455) -> (index of element=w454:i32)  [unwired: 1 in]
                        n367 = Greater Or Equal To 0?(x=w454) -> (x >= 0?=w452:bool)
                        n368 = Replace Array Subset(array=w450, new element=TRUE ("nouvel élément/sous-tableau"), index=w454) -> (w451:bool[])
                        n369 = Select(t=w451, s=w452, f=w450) -> (s? t:f=w449:bool[])
                      }
                      n370 = local write "Selection EDWARDS"(w445) -> ()
                    }
                  }
                }
              }
            }
            event "Th n°": Value Change {
              n371 = event-data() -> ()  [unwired: 1 in, 5 out]
              n372 = global read "Variable glob Th.vi" "Taches Th"() -> (w458:T13)
              n373 = for {
                tunnel: w458 -> [w465] mode=indexing
                tunnel: [w464] -> w457 mode=indexing
                n374 = Unbundle By Name(w465) -> ("Nom tache Th"=w464:refnum<k21>)
              }
              n375 = Decrement(x="Th n°") -> (x-1=w462:u8)
              n376 = Build Array(w462) -> (w461:u8[])
              n377 = Index Array(array=w457, index=w462) -> (element=w463:refnum<k21>)
              n378 = property on="Tableau Th" class="Tabl (strict)"("Index Values"=w461) -> (error out=w459:errorcluster)  [unwired: 2 in, 1 out]
              n379 = local write "Nom de la tache Th associee"(w463) -> ()
              n380 = call <vilib>:"Clear Errors.vi"("error in (no error)"=w459) -> ()  [unwired: 5 in, 2 out]
            }
            event "Pt n°": Value Change {
              n381 = event-data() -> ()  [unwired: 1 in, 5 out]
              n382 = global read "Variable glob Pt.vi" "Taches Pt 100"() -> (w467:T15)
              n383 = for {
                tunnel: w467 -> [w474] mode=indexing
                tunnel: [w473] -> w466 mode=indexing
                n384 = Unbundle By Name(w474) -> ("Nom tache Pt"=w473:refnum<k21>)
              }
              n385 = Decrement(x="Pt n°") -> (x-1=w471:u8)
              n386 = Build Array(w471) -> (w470:u8[])
              n387 = property on="Tableau Pt" class="Tabl (strict)"("Index Values"=w470) -> (error out=w468:errorcluster)  [unwired: 2 in, 1 out]
              n388 = Index Array(array=w466, index=w471) -> (element=w472:refnum<k21>)
              n389 = call <vilib>:"Clear Errors.vi"("error in (no error)"=w468) -> ()  [unwired: 5 in, 2 out]
              n390 = local write "Nom de la tache Pt associee"(w472) -> ()
            }
            event "Port COM REG": Value Change {
              n391 = event-data() -> ("NewVal"=w477:u16)  [unwired: 1 in, 5 out]
              n392 = Build Array(w477, u16 0 ("élément")) -> (w475:u16[])
              n393 = property on="Reg dispo" class="Tabl (strict)"("Index Values"=w475) -> ()  [unwired: 2 in, 2 out]
              n394 = property on="Donnees reg" class="Tabl (strict)"("Index Values"=w475) -> ()  [unwired: 2 in, 2 out]
            }
            event "Init compteurs (m3)", "Temps pour débit": Value Change {
              n395 = event-data() -> ()  [unwired: 1 in, 6 out]
              n396 = local read "Init compteurs (m3)"() -> (w478:dbl[])
              n397 = global read "Variable globale compteurs.vi" "Tache Compteurs"() -> (w481:T19)
              n398 = local read "Selection"() -> (w479:bool[])
              n399 = Bundle By Name(cluster=w481, "Selection"=w479, "Init compteurs"=w478) -> (w480:T19)
              n400 = global write "Variable globale compteurs.vi" "Tache Compteurs"(w480) -> ()
            }
            event "Experiences precedentes": Value Change {
              n401 = event-data() -> ("NewVal"=w492:u16)  [unwired: 1 in, 1 out]
              n402 = global read "Variable glob generale.vi" "Dossier cuve local"() -> (w494:path)
              n403 = property on="Experiences precedentes" class="MDér (strict)"() -> ("Strings []"=w493:string[])  [unwired: 2 in, 2 out]
              n404 = Index Array(array=w493, index=w492) -> (element=w484:string)
              n405 = Build Path(base path=w494, name or relative path=w484) -> (appended path=w491:path)
              n406 = local write "Nom manip"(w484) -> ()
              n407 = List Folder(path=w491) -> (folder names=w497:string[])  [unwired: 3 in, 3 out]
              n408 = for {
                tunnel: w497 -> [w522] mode=indexing
                shift-right: [w520] -> w503
                shift-left: string[] [] -> [w519]
                n409 = Decimal String To Number(string=w522) -> (number=w524:i32)  [unwired: 2 in, 1 out]
                n410 = Build Array (concatenate)(w519, w522) -> (w521:string[])
                n411 = Equal To 0?(x=w524) -> (x = 0?=w523:bool)
                n412 = Select(t=w521, s=w523, f=w519) -> (s? t:f=w520:string[])
              }
              n413 = global read "Variable glob generale.vi" "Dossier cuve distant"() -> (w486:path)
              n414 = Array Size(array=w503) -> (size(s)=w498:i32)
              n415 = Equal?(x=w486, y=path "") -> (x = y?=w487:bool)
              n416 = Build Array (concatenate)("", w503) -> (w500:string[])
              n417 = Not Equal To 0?(x=w498) -> (x != 0?=w499:bool)
              n418 = Select(t=w500, s=w499, f=w503) -> (s? t:f=w501:string[])
              n419 = Index Array(array=w501, index=0 ("indice")) -> (element=w483:string)
              n420 = Equal?(x=w483, y="") -> (x = y?=w482:bool)
              n421 = case shown="Faux" w487 {
                tunnel: w486 -> [w508 w514]
                tunnel: [w505 w514] -> w485
                tunnel: w484 -> [w509 _]
                tunnel: w483 -> [w506 _]
                tunnel: w482 -> [w504 _]
                frame False {
                  n422 = Build Path(base path=w508, name or relative path=w509) -> (appended path=w507:path)
                  n423 = case shown="Faux" w504 {
                    tunnel: w507 -> [w512 w513]
                    tunnel: w506 -> [w511 _]
                    tunnel: [w510 w513] -> w505
                    frame False {
                      n424 = Build Path(base path=w512, name or relative path=w511) -> (appended path=w510:path)
                    }
                    frame True {
                    }
                  }
                }
                frame True {
                }
              }
              n425 = property on="Sous-dossier precedents" class="MDér (strict)"("Strings []"=w501) -> ()  [unwired: 2 in, 2 out]
              n426 = case shown="Faux" w482 {
                tunnel: w491 -> [w517 w518]
                tunnel: w483 -> [w516 _]
                tunnel: [w515 w518] -> w490
                frame False {
                  n427 = Build Path(base path=w517, name or relative path=w516) -> (appended path=w515:path)
                }
                frame True {
                }
              }
              n428 = local write "Sous-dossier eventuel"(w483) -> ()
              n429 = local write "Chemin DATA local"(w490) -> ()
              n430 = local write "Chemin DATA distant"(w485) -> ()
            }
            event "Nom manip": Value Change {
              n431 = event-data() -> ("NewVal"=w531:string)  [unwired: 1 in, 5 out]
              n432 = global read "Variable glob generale.vi" "Dossier cuve distant"() -> (w526:path)
              n433 = global read "Variable glob generale.vi" "Dossier cuve local"() -> (w535:path)
              n434 = local read "Sous-dossier eventuel"() -> (w529:string)
              n435 = Equal?(x=path "", y=w526) -> (x = y?=w527:bool)
              n436 = Build Path(base path=w535, name or relative path=w531) -> (appended path=w532:path)
              n437 = Equal?(x=w529, y="") -> (x = y?=w528:bool)
              n438 = case shown="Faux" w527 {
                tunnel: w526 -> [w541 w546]
                tunnel: w531 -> [w540 _]
                tunnel: [w539 w546] -> w530
                tunnel: w529 -> [w537 _]
                tunnel: w528 -> [w536 _]
                frame False {
                  n439 = Build Path(base path=w541, name or relative path=w540) -> (appended path=w538:path)
                  n440 = case shown="Faux" w536 {
                    tunnel: w538 -> [w544 w545]
                    tunnel: w537 -> [w543 _]
                    tunnel: [w542 w545] -> w539
                    frame False {
                      n441 = Build Path(base path=w544, name or relative path=w543) -> (appended path=w542:path)
                    }
                    frame True {
                    }
                  }
                }
                frame True {
                }
              }
              n442 = case shown="Faux" w528 {
                tunnel: w532 -> [w549 w550]
                tunnel: w529 -> [w548 _]
                tunnel: [w547 w550] -> w533
                frame False {
                  n443 = Build Path(base path=w549, name or relative path=w548) -> (appended path=w547:path)
                }
                frame True {
                }
              }
              n444 = local write "Chemin DATA local"(w533) -> ()
              n445 = local write "Chemin DATA distant"(w530) -> ()
            }
            event "Sous-dossier precedents": Value Change {
              n446 = event-data() -> ("NewVal"=w562:u16)  [unwired: 1 in, 5 out]
              n447 = local read "Nom manip"() -> (w553:string)
              n448 = global read "Variable glob generale.vi" "Dossier cuve distant"() -> (w555:path)
              n449 = global read "Variable glob generale.vi" "Dossier cuve local"() -> (w561:path)
              n450 = property on="Sous-dossier precedents" class="MDér (strict)"() -> ("Strings []"=w563:string[])  [unwired: 2 in, 2 out]
              n451 = Index Array(array=w563, index=w562) -> (element=w551:string)
              n452 = Build Path(base path=w561, name or relative path=w553) -> (appended path=w559:path)
              n453 = Equal?(x=path "", y=w555) -> (x = y?=w556:bool)
              n454 = local write "Sous-dossier eventuel"(w551) -> ()
              n455 = Equal?(x=w551, y="") -> (x = y?=w552:bool)
              n456 = case shown="Faux" w556 {
                tunnel: w555 -> [w569 w574]
                tunnel: w553 -> [w568 _]
                tunnel: [w567 w574] -> w557
                tunnel: w552 -> [w565 _]
                tunnel: w551 -> [w564 _]
                frame False {
                  n457 = Build Path(base path=w569, name or relative path=w568) -> (appended path=w566:path)
                  n458 = case shown="Faux" w565 {
                    tunnel: w566 -> [w572 w573]
                    tunnel: w564 -> [w571 _]
                    tunnel: [w570 w573] -> w567
                    frame False {
                      n459 = Build Path(base path=w572, name or relative path=w571) -> (appended path=w570:path)
                    }
                    frame True {
                    }
                  }
                }
                frame True {
                }
              }
              n460 = case shown="Faux" w552 {
                tunnel: [w577 w578] -> w560
                tunnel: w559 -> [w576 w578]
                tunnel: w551 -> [w575 _]
                frame False {
                  n461 = Build Path(base path=w576, name or relative path=w575) -> (appended path=w577:path)
                }
                frame True {
                }
              }
              n462 = local write "Chemin DATA distant"(w557) -> ()
              n463 = local write "Chemin DATA local"(w560) -> ()
            }
            event "Sous-dossier eventuel": Value Change {
              n464 = event-data() -> ()  [unwired: 1 in, 6 out]
              n465 = local read "Nom manip"() -> (w581:string)
              n466 = global read "Variable glob generale.vi" "Dossier cuve distant"() -> (w583:path)
              n467 = local read "Sous-dossier eventuel"() -> (w579:string)
              n468 = global read "Variable glob generale.vi" "Dossier cuve local"() -> (w589:path)
              n469 = Equal?(x=path "", y=w583) -> (x = y?=w584:bool)
              n470 = Build Path(base path=w589, name or relative path=w581) -> (appended path=w586:path)
              n471 = Equal?(x=w579, y="") -> (x = y?=w580:bool)
              n472 = case shown="Faux" w584 {
                tunnel: w583 -> [w595 w600]
                tunnel: w581 -> [w594 _]
                tunnel: [w593 w600] -> w585
                tunnel: w580 -> [w591 _]
                tunnel: w579 -> [w590 _]
                frame False {
                  n473 = Build Path(base path=w595, name or relative path=w594) -> (appended path=w592:path)
                  n474 = case shown="Faux" w591 {
                    tunnel: w592 -> [w598 w599]
                    tunnel: w590 -> [w597 _]
                    tunnel: [w596 w599] -> w593
                    frame False {
                      n475 = Build Path(base path=w598, name or relative path=w597) -> (appended path=w596:path)
                    }
                    frame True {
                    }
                  }
                }
                frame True {
                }
              }
              n476 = case shown="Faux" w580 {
                tunnel: w586 -> [w603 w604]
                tunnel: w579 -> [w602 _]
                tunnel: [w601 w604] -> w588
                frame False {
                  n477 = Build Path(base path=w603, name or relative path=w602) -> (appended path=w601:path)
                }
                frame True {
                }
              }
              n478 = local write "Chemin DATA local"(w588) -> ()
              n479 = local write "Chemin DATA distant"(w585) -> ()
            }
            event "Commentaire dans le fichier :": Mouse Down {
              n480 = event-data() -> ()  [unwired: 1 in, 8 out]
              n481 = property on="Commentaire dans le fichier :" class="Ch"("Text.BGColor"=u32 16777215) -> ()  [unwired: 2 in, 2 out]
            }
            event "Chemin DATA distant": Value Change {
              n482 = event-data() -> ("NewVal"=w607:path)  [unwired: 1 in, 4 out]
              n483 = Not Equal?(x=w607, y=path "") -> (x != y?=w609:bool)
              n484 = case shown="Vrai" w609 {
                tunnel: w607 -> [w610 w618]
                tunnel: [w610 w613] -> w606
                frame False {
                }
                frame True {
                  n485 = disable-structure shown="Désactivé" {
                    disable-tunnel: w618 -> [w621 w622]
                    disable-tunnel: [w620 w622] -> w617
                    frame Disabled {
                      n486 = local read "CUVE"() -> (w619:string)
                      n487 = Build Path(base path=w621, name or relative path=w619) -> (appended path=w620:path)
                    }
                    frame Enabled {
                    }
                  }
                  n488 = local read "Sous-dossier eventuel"() -> (w612:string)
                  n489 = local read "Nom manip"() -> (w611:string)
                  n490 = Build Path(base path=w617, name or relative path=w611) -> (appended path=w614:path)
                  n491 = Not Equal?(x="", y=w612) -> (x != y?=w616:bool)
                  n492 = case shown="Vrai" w616 {
                    tunnel: w612 -> [_ w626]
                    tunnel: w614 -> [w623 w625]
                    tunnel: [w623 w624] -> w613
                    frame False {
                    }
                    frame True {
                      n493 = Build Path(base path=w625, name or relative path=w626) -> (appended path=w624:path)
                    }
                  }
                }
              }
              n494 = local write "Chemin DATA distant"(w606) -> ()
            }
          }
        }
        n495 = Select(t=Enum_3."arret acquisitions" ("Énum"), s=w344, f=Enum_3."enregistrement var glob pres" ("Énum")) -> (s? t:f=w342:T6)
      }
      frame "enregistrement var glob pres" {
        # "Envoi du choix dans les variables globales"
        n496 = global write "Variable glob Edwards.vi" "Noms Edwards"("Nom des jauges EDWARDS") -> ()
        n497 = global write "Variable glob Edwards.vi" "Select Edwards"("Selection EDWARDS") -> ()
        n498 = Array Size(array="Selection EDWARDS") -> (size(s)=w651:i32[])
        n499 = global write "Variable glob Leybold.vi" "Selection Leybold"("Selection\nLEYBOLD") -> ()
        n500 = global write "Variable glob Keller.vi" "Selection KELLER"("Selection\nKELLER") -> ()
        n501 = global write "Variable glob Keller.vi" "Noms KELLER"("Nom des jauges KELLER") -> ()
        n502 = Index Array(array=w651, index=0 ("indice")) -> (element=w648:i32)
        n503 = Index Array(array=w651, index=1 ("indice")) -> (element=w647:i32)
        n504 = global write "Variable glob Leybold.vi" "Noms Leybold"("Nom des jauges\nLEYBOLD") -> ()
        n505 = Transpose 2D Array(2D array="Nom des jauges EDWARDS") -> (transposed array=w659:string[][])
        n506 = Transpose 2D Array(2D array="Selection EDWARDS") -> (transposed array=w658:bool[][])
        n507 = Initialize Array("", 0 ("taille de la dimension")) -> (w660:string[])
        n508 = Multiply(x=w648, y=w647) -> (x*y=w657:i32)
        n509 = Initialize Array("", 0 ("taille de la dimension")) -> (w645:string[])
        n510 = Reshape Array(w658, w657) -> (w655:bool[])
        n511 = Reshape Array(w659, w657) -> (w656:string[])
        n512 = for {
          tunnel: "Nom des jauges\nLEYBOLD" -> [w682] mode=indexing
          tunnel: "Selection\nLEYBOLD" -> [w683] mode=indexing
          shift-right: [w680] -> w646
          shift-left: w660 -> [w681]
          n513 = case shown="Vrai" w683 {
            tunnel: w682 -> [_ w687]
            tunnel: w681 -> [w684 w686]
            tunnel: [w684 w685] -> w680
            frame False {
            }
            frame True {
              n514 = Build Array (concatenate)(w686, w687) -> (w685:string[])
            }
          }
        }
        n515 = Initialize Array("", 0 ("taille de la dimension")) -> (w654:string[])
        n516 = for {
          tunnel: "Nom des jauges KELLER" -> [w674] mode=indexing
          tunnel: "Selection\nKELLER" -> [w675] mode=indexing
          shift-right: [w672] -> w642
          shift-left: w645 -> [w673]
          n517 = case shown="Vrai" w675 {
            tunnel: w674 -> [_ w679]
            tunnel: w673 -> [w676 w678]
            tunnel: [w676 w677] -> w672
            frame False {
            }
            frame True {
              n518 = Build Array (concatenate)(w678, w679) -> (w677:string[])
            }
          }
        }
        n519 = for {
          tunnel: w656 -> [w690] mode=indexing
          tunnel: w655 -> [w691] mode=indexing
          shift-right: [w688] -> w663
          shift-left: w654 -> [w689]
          n520 = case shown="Vrai" w691 {
            tunnel: w690 -> [_ w695]
            tunnel: w689 -> [w692 w694]
            tunnel: [w692 w693] -> w688
            frame False {
            }
            frame True {
              n521 = Build Array (concatenate)(w694, w695) -> (w693:string[])
            }
          }
        }
        n522 = global write "Variable glob Leybold.vi" "Nom select Leybold"(w646) -> ()
        n523 = global write "Variable glob Edwards.vi" "Nom select Edwards"(w663) -> ()
        n524 = global write "Variable glob Keller.vi" "Noms KELLER selectionnes"(w642) -> ()
        n525 = Index Array(array="Grappes", index (col)=0 ("indice désactivé (col)")) -> (element=w629:string[])  [unwired: 1 in]
        n526 = Initialize Array("", 0 ("taille de la dimension")) -> (w632:string[])
        n527 = global write "Variable glob Edwards.vi" "Select Grappes"("Selection\nGrappes") -> ()
        n528 = for {
          tunnel: w629 -> [w666] mode=indexing
          tunnel: "Selection\nGrappes" -> [w667] mode=indexing
          shift-right: [w664] -> w628
          shift-left: w632 -> [w665]
          n529 = case shown="Vrai" w667 {
            tunnel: w666 -> [_ w671]
            tunnel: w665 -> [w668 w670]
            tunnel: [w668 w669] -> w664
            frame False {
            }
            frame True {
              n530 = Build Array (concatenate)(w670, w671) -> (w669:string[])
            }
          }
        }
        n531 = global write "Variable glob Edwards.vi" "Nom select grappes"(w628) -> ()
      }
      frame "enregistrement var glob temp" {
        n532 = local read "Tableau Th"() -> (w699:T2)
        n533 = global read "Variable glob Th.vi" "Taches Th"() -> (w700:T13)
        n534 = global read "Variable glob Pt.vi" "Taches Pt 100"() -> (w704:T15)
        n535 = local read "Tableau Pt"() -> (w706:T3)
        n536 = for {
          tunnel: w699 -> [w716] mode=indexing
          tunnel: w700 -> [w714] mode=indexing
          tunnel: [w713] -> w696 mode=indexing
          tunnel: [w707] -> w698 mode=concatenating
          n537 = Unbundle By Name(w716) -> ("Noms Thermocouples :"=w715:string[], "Selection Th"=w707:bool[])
          n538 = for {
            tunnel: w715 -> [w729] mode=indexing
            tunnel: [w725] -> w712 mode=indexing
            n539 = Search and Replace String(replace all?=TRUE ("tout remplacer ? (F)"), input string=w729, search string="\r\n", replace string="") -> (result string=w725:string)  [unwired: 4 in, 3 out]
          }
          n540 = Initialize Array("", 0 ("taille de la dimension")) -> (w709:string[])
          n541 = for {
            tunnel: w712 -> [w719] mode=indexing
            tunnel: w707 -> [w718] mode=indexing
            shift-right: [w717] -> w708
            shift-left: w709 -> [w720]
            n542 = case shown="Vrai" w718 {
              tunnel: w720 -> [w721 w724]
              tunnel: [w721 w723] -> w717
              tunnel: w719 -> [_ w722]
              frame False {
              }
              frame True {
                n543 = Build Array (concatenate)(w724, w722) -> (w723:string[])
              }
            }
          }
          n544 = Bundle By Name(cluster=w714, "Nom Th selectionnes"=w708, "Noms des Th"=w712, "Selection Th"=w707) -> (w713:T21)
        }
        n545 = for {
          tunnel: w706 -> [w739] mode=indexing
          tunnel: w704 -> [w737] mode=indexing
          tunnel: [w736] -> w703 mode=indexing
          tunnel: [w730] -> w702 mode=concatenating
          n546 = Unbundle By Name(w739) -> ("Noms Platines :"=w738:string[], "Sélection Pt"=w730:bool[])
          n547 = for {
            tunnel: w738 -> [w752] mode=indexing
            tunnel: [w748] -> w735 mode=indexing
            n548 = Search and Replace String(replace all?=TRUE ("tout remplacer ? (F)"), input string=w752, search string="\r\n", replace string="") -> (result string=w748:string)  [unwired: 4 in, 3 out]
          }
          n549 = Initialize Array("", 0 ("taille de la dimension")) -> (w732:string[])
          n550 = for {
            tunnel: w735 -> [w742] mode=indexing
            tunnel: w730 -> [w741] mode=indexing
            shift-right: [w740] -> w731
            shift-left: w732 -> [w743]
            n551 = case shown="Vrai" w741 {
              tunnel: w743 -> [w744 w747]
              tunnel: [w744 w746] -> w740
              tunnel: w742 -> [_ w745]
              frame False {
              }
              frame True {
                n552 = Build Array (concatenate)(w747, w745) -> (w746:string[])
              }
            }
          }
          n553 = Bundle By Name(cluster=w737, "Nom Pt selectionnees"=w731, "Noms des Pt"=w735, "Selection Pt"=w730) -> (w736:T22)
        }
        n554 = Or Array Elements(Boolean array=w702) -> (logical OR=w701:bool)
        n555 = Or Array Elements(Boolean array=w698) -> (logical OR=w697:bool)
        n556 = global write "Variable glob Pt.vi" "Taches Pt 100"(w703) -> ()
        n557 = global write "Variable glob Th.vi" "Taches Th"(w696) -> ()
        n558 = global write "Variable glob Pt.vi" "Temp Pt"(w701) -> ()
        n559 = global write "Variable glob Th.vi" "Temp Th"(w697) -> ()
      }
      frame "enregistrement var glob reg" {
        n560 = for {
          tunnel: "Reg dispo" -> [w834] mode=indexing
          tunnel: [w828] -> w768 mode=indexing
          tunnel: [w830] -> w767 mode=indexing
          tunnel: [w832] -> w769 mode=indexing
          tunnel: [w827] -> w754 mode=indexing
          n561 = Unbundle By Name(w834) -> ("1 COM reg"=w833:T8)
          n562 = for {
            tunnel: w833 -> [w838] mode=indexing
            tunnel: [w837] -> w829 mode=indexing
            tunnel: [w836] -> w831 mode=indexing
            tunnel: [w835] -> w827 mode=indexing
            n563 = Unbundle By Name(w838) -> ("Nom"=w837:string, "Adresse"=w836:u8, "sélect"=w835:bool)
          }
          n564 = Bundle(w827) -> (w832:cluster{bool[]})  [unwired: 1 in]
          n565 = Bundle(w831) -> (w830:cluster{u8[]})  [unwired: 1 in]
          n566 = Bundle(w829) -> (w828:cluster{string[]})  [unwired: 1 in]
        }
        n567 = global read "Variables glob EUROTHERM.vi" "Ports COM REG dispo"() -> (w765:refnum<visa-resource-name>[])
        n568 = Or Array Elements(Boolean array=w754) -> (logical OR=w753:bool)
        n569 = global write "Variables glob EUROTHERM.vi" "REG"(w753) -> ()
        n570 = global write "Variables glob EUROTHERM.vi" "Select regs acqui"(w769) -> ()
        n571 = for {
          tunnel: w769 -> [w786] mode=indexing
          tunnel: w768 -> [w788] mode=indexing
          tunnel: w767 -> [w785] mode=indexing
          tunnel: w765 -> [w781] mode=indexing
          shift-right: [w779] -> w763
          shift-left: refnum<visa-resource-name>[] [] -> [w780]
          shift-right: [w778] -> w762
          shift-left: cluster{string[]}[] [] -> [w777]
          shift-right: [w775] -> w761
          shift-left: cluster{u8[]}[] [] -> [w776]
          shift-right: [w771] -> w756
          shift-left: cluster{bool[]}[] [] -> [w772]
          shift-right: [w773] -> w757
          shift-left: i32[] [] -> [w774]
          # "chaque COM dispo"
          n572 = Unbundle(w785) -> (w784:u8[])
          n573 = Unbundle(w786) -> (w783:bool[])
          n574 = Unbundle(w788) -> (w787:string[])
          n575 = Or Array Elements(Boolean array=w783) -> (logical OR=w782:bool)
          n576 = case shown="Vrai" w782 {
            tunnel: w787 -> [_ w815]
            tunnel: w784 -> [_ w814]
            tunnel: w783 -> [_ w810]
            tunnel: w781 -> [_ w807]
            tunnel: w780 -> [w793 w808]
            tunnel: [w793 w806] -> w779
            tunnel: [w792 w804] -> w778
            tunnel: w777 -> [w792 w803]
            tunnel: w776 -> [w791 w801]
            tunnel: [w791 w800] -> w775
            tunnel: w774 -> [w790 w798]
            tunnel: [w790 w797] -> w773
            tunnel: w772 -> [w789 w796]
            tunnel: [w789 w794] -> w771
            frame False {
            }
            frame True {
              n577 = Build Array (concatenate)(w808, w807) -> (w806:refnum<visa-resource-name>[])
              n578 = for {
                tunnel: w810 -> [w820] mode=indexing
                shift-right: [w825] -> w809
                shift-left: string[] [] -> [w818]
                tunnel: w814 -> [w821] mode=indexing
                shift-right: [w823] -> w813
                shift-left: u8[] [] -> [w822]
                tunnel: w815 -> [w819] mode=indexing
                # "chaque reg"
                n579 = Build Array (concatenate)(w822, w821) -> (w824:u8[])
                n580 = Build Array (concatenate)(w818, w819) -> (w826:string[])
                n581 = Select(t=w826, s=w820, f=w818) -> (s? t:f=w825:string[])
                n582 = Select(t=w824, s=w820, f=w822) -> (s? t:f=w823:u8[])
              }
              n583 = Array Size(array=w813) -> (size(s)=w799:i32)
              n584 = Bundle(w809) -> (w805:cluster{string[]})  [unwired: 1 in]
              n585 = Bundle(w813) -> (w802:cluster{u8[]})  [unwired: 1 in]
              n586 = Initialize Array(TRUE, w799) -> (w811:bool[])
              n587 = Build Array (concatenate)(w798, w799) -> (w797:i32[])
              n588 = Bundle(w811) -> (w795:cluster{bool[]})  [unwired: 1 in]
              n589 = Build Array (concatenate)(w803, w805) -> (w804:cluster{string[]}[])
              n590 = Build Array (concatenate)(w801, w802) -> (w800:cluster{u8[]}[])
              n591 = Build Array (concatenate)(w796, w795) -> (w794:cluster{bool[]}[])
            }
          }
        }
        n592 = global write "Variables glob EUROTHERM.vi" "Ports COM REG acqui"(w763) -> ()
        n593 = global write "Variables glob EUROTHERM.vi" "Nb reg acqui"(w757) -> ()
        n594 = global write "Variables glob EUROTHERM.vi" "Noms voies regs select acqui"(w762) -> ()
        n595 = global write "Variables glob EUROTHERM.vi" "Adresses regs acqui"(w761) -> ()
        n596 = global write "Variables glob EUROTHERM.vi" "Select regs run"(w756) -> ()
      }
      frame "enregistrement var glob compt et dossiers" {
        n597 = local read "Noms des compteurs"() -> (w854:string[])
        n598 = global write "Variable glob generale.vi" "Dossier sauvegarde"("Chemin sauvegarde") -> ()
        n599 = global write "Variable glob generale.vi" "Commentaire"("Commentaire dans le fichier :") -> ()
        n600 = for {
          tunnel: w854 -> [w890] mode=indexing
          tunnel: "Selection" -> [w891] mode=indexing
          shift-right: [w888] -> w851
          shift-left: string[] [] -> [w887]
          n601 = Build Array (concatenate)(w887, w890) -> (w889:string[])
          n602 = Select(t=w889, s=w891, f=w887) -> (s? t:f=w888:string[])
        }
        n603 = local read "Nom manip"() -> (w848:string)
        n604 = local read "Chemin DATA distant"() -> (w842:path)
        n605 = local read "Chemin DATA local"() -> (w846:path)
        n606 = Equal?(x="", y=w848) -> (x = y?=w840:bool)
        n607 = global write "Variable glob generale.vi" "Sous-dossier"("Sous-dossier eventuel") -> ()
        n608 = global write "Variable glob generale.vi" "Nom manip"(w848) -> ()
        n609 = global read "Variable globale compteurs.vi" "Tache Compteurs"() -> (w858:T19)
        n610 = Bundle By Name(cluster=w858, "Noms des compteurs"=w854, "Selection"="Selection", "Init compteurs"="Init compteurs (m3)", "Noms compteurs selectionnes"=w851) -> (w856:T19)
        n611 = Equal?(x=w842, y=path "") -> (x = y?=w843:bool)
        n612 = case shown="Faux" w840 {
          tunnel: w846 -> [w877 w886]
          tunnel: [w876 w886] -> w845
          tunnel: "Sous-dossier eventuel" -> [w880 _]
          frame False {
            n613 = Equal?(x="", y=w880) -> (x = y?=w878:bool)
            n614 = case shown="Faux" w878 {
              tunnel: w877 -> [w883 w885]
              tunnel: [w881 w884] -> w876
              frame False {
                n615 = Strip Path(path=w883) -> (stripped path=w882:path)  [unwired: 1 out]
                n616 = Strip Path(path=w882) -> (stripped path=w881:path)  [unwired: 1 out]
              }
              frame True {
                n617 = Strip Path(path=w885) -> (stripped path=w884:path)  [unwired: 1 out]
              }
            }
          }
          frame True {
          }
        }
        n618 = case shown="Faux" w843 {
          tunnel: w842 -> [w862 w875]
          tunnel: [w861 w875] -> w841
          tunnel: w840 -> [w863 _]
          tunnel: "Sous-dossier eventuel" -> [w860 _]
          frame False {
            n619 = case shown="Faux" w863 {
              tunnel: w862 -> [w865 w874]
              tunnel: [w864 w874] -> w861
              tunnel: w860 -> [w866 _]
              frame False {
                n620 = Equal?(x="", y=w866) -> (x = y?=w868:bool)
                n621 = case shown="Faux" w868 {
                  tunnel: w865 -> [w871 w873]
                  tunnel: [w869 w872] -> w864
                  frame False {
                    n622 = Strip Path(path=w871) -> (stripped path=w870:path)  [unwired: 1 out]
                    n623 = Strip Path(path=w870) -> (stripped path=w869:path)  [unwired: 1 out]
                  }
                  frame True {
                    n624 = Strip Path(path=w873) -> (stripped path=w872:path)  [unwired: 1 out]
                  }
                }
              }
              frame True {
              }
            }
          }
          frame True {
          }
        }
        n625 = global write "Variable globale compteurs.vi" "Temps débit"("Temps pour débit") -> ()
        n626 = global write "Variable globale compteurs.vi" "Tache Compteurs"(w856) -> ()
        n627 = global write "Variable glob generale.vi" "Dossier cuve local"(w845) -> ()
        n628 = global write "Variable glob generale.vi" "Dossier cuve distant"(w841) -> ()
      }
      frame "creation dossiers" {
        n629 = global read "Variable glob generale.vi" "Dossier sauvegarde"() -> (w906:path)
        n630 = global read "Variable glob generale.vi" "Dossier cuve distant"() -> (w903:path)
        n631 = global read "Variable glob generale.vi" "Dossier cuve local"() -> (w895:path)
        n632 = Not Equal?(x=w906, y=path "") -> (x != y?=w904:bool)
        n633 = Not Equal?(x=w903, y=path "") -> (x != y?=w902:bool)
        n634 = case shown="Vrai" w904 {
          tunnel: w906 -> [_ w910]
          tunnel: [errorcluster {"status"=FALSE, "code"=0, "source"=""} ("error out") w909] -> w893
          frame False {
          }
          frame True {
            n635 = call <vilib>:"Check if File or Folder Exists.vi"("path"=w910) -> ("error out"=w913:errorcluster, "file or folder exists?"=w911:bool, "dup path"=w912:path)  [unwired: 8 in]
            n636 = case shown="Faux" w911 {
              tunnel: w912 -> [w916 _]
              tunnel: w913 -> [w915 w917]
              tunnel: [w914 w917] -> w909
              frame False {
                n637 = Create Folder(path (use dialog)=w916, error in=w915) -> (error out=w914:errorcluster)  [unwired: 1 in, 2 out]
              }
              frame True {
              }
            }
          }
        }
        n638 = case shown="Vrai" w902 {
          tunnel: w903 -> [_ w920]
          tunnel: [errorcluster {"status"=FALSE, "code"=0, "source"=""} ("error out") w919] -> w894
          frame False {
          }
          frame True {
            n639 = call <vilib>:"Check if File or Folder Exists.vi"("path"=w920) -> ("error out"=w923:errorcluster, "file or folder exists?"=w921:bool, "dup path"=w922:path)  [unwired: 8 in]
            n640 = case shown="Faux" w921 {
              tunnel: w922 -> [w926 _]
              tunnel: w923 -> [w925 w927]
              tunnel: [w924 w927] -> w919
              frame False {
                n641 = Create Folder(path (use dialog)=w926, error in=w925) -> (error out=w924:errorcluster)  [unwired: 1 in, 2 out]
              }
              frame True {
              }
            }
          }
        }
        n642 = call <vilib>:"Check if File or Folder Exists.vi"("path"=w895) -> ("error out"=w898:errorcluster, "file or folder exists?"=w896:bool, "dup path"=w897:path)  [unwired: 8 in]
        n643 = case shown="Faux" w896 {
          tunnel: w897 -> [w931 _]
          tunnel: w898 -> [w930 w932]
          tunnel: [w929 w932] -> w899
          frame False {
            n644 = Create Folder(path (use dialog)=w931, error in=w930) -> (error out=w929:errorcluster)  [unwired: 1 in, 2 out]
          }
          frame True {
          }
        }
        n645 = Merge Errors(w899, w894, w893) -> (w900:errorcluster)
        n646 = case shown="Erreur" w900 {
          tunnel: "Erreur lors de la création de l'un des dossiers.\nPour le dossier distant et le dossier de sauvegarde, vérifier que la connection réseau est possible avec l'explorateur Windows" -> [_ w928]
          frame No Error {
          }
          frame Error {
            n647 = One Button Dialog(message=w928) -> ()  [unwired: 1 in, 1 out]
          }
        }
      }
      frame "enregistrement fichier config" {
        n648 = Build Path(base path=path "C:/LABVIEW/PRES+TEMP+REG dernière version/Configurations", name or relative path="config acqui.ini" ("nom ou chemin relatif")) -> (appended path=w956:path)
        n649 = call <vilib>:"Open Config Data.vi"("create file if necessary (T)"=TRUE ("create file if necessary? (T)"), "configuration file path"=w956) -> ("error out"=w953:errorcluster, "refnum"=w954:T23)  [unwired: 7 in, 1 out]
        n650 = call "Ecrire config gene.vi"("error in (no error)"=w953, "refnum"=w954) -> ("error out"=w952:errorcluster, "refnum out"=w951:T23)
        n651 = call "Ecrire config LEYBOLD.vi"("error in (no error)"=w952, "refnum"=w951) -> ("error out"=w950:errorcluster, "refnum out"=w949:T23)
        n652 = global write "Variable glob generale.vi" "Config OK"(TRUE ("Config OK")) -> ()
        n653 = call "Ecrire config EDWARDS.vi"("error in (no error)"=w950, "refnum"=w949) -> ("error out"=w948:errorcluster, "refnum out"=w947:T23)
        n654 = call "Ecrire config KELLER.vi"("error in (no error)"=w948, "refnum"=w947) -> ("error out"=w946:errorcluster, "refnum out"=w945:T23)
        n655 = call "Ecrire config Th.vi"("error in (no error)"=w946, "refnum"=w945) -> ("error out"=w944:errorcluster, "refnum out"=w943:T23)
        n656 = call "Ecrire config.vi"("error in (no error)"=w944, "refnum"=w943) -> ("error out"=w938:errorcluster, "refnum out"=w939:T23)
        n657 = call "Ecrire config REG.vi"("error in (no error) 2"=w938, "refnum 2"=w939) -> ("error out"=w935:errorcluster, "refnum out"=w936:T23)
        n658 = call "Ecrire config compteurs.vi"("error in (no error)"=w935, "refnum"=w936) -> ("error out"=w933:errorcluster, "refnum out"=w934:T23)
        n659 = call <vilib>:"Close Config Data.vi"("error in (no error)"=w933, "refnum"=w934) -> ("error out"=w940:errorcluster)  [unwired: 8 in, 1 out]
        n660 = call <vilib>:"Clear Errors.vi"("error in (no error)"=w940) -> ()  [unwired: 5 in, 2 out]
      }
      frame "arret acquisitions" {
        w959 = FALSE ("Lancement")
        # "Arret de l'acquisition de l'ensemble des voies"
        n661 = call "Arret acquisitions.vi"() -> ()  [unwired: 12 in]
        n662 = global write "Variable glob generale.vi" "Lancement"(w959) -> ()
        n663 = global write "Variable glob generale.vi" "Acqui tout"(w959) -> ()
      }
      frame "fin" {
        n664 = flat-sequence {
          frame #0 {
            # "Réouverture face avant programme principal"
            n665 = local read "sortie d'erreur"() -> (w963:errorcluster)
            n666 = local read "Refnum VI"() -> (w964:refnum<vi>)
            n667 = invoke class="VI" method="FA.Ouvrir"(reference=w964, error in=w963, "Activate"=TRUE ("Activer ?"), "State"=T10."Standard" ("État")) -> (reference out=w967:refnum<vi>, error out=w968:errorcluster)  [unwired: 1 in, 3 out]
            n668 = Close Reference(reference=w967, error in (no error)=w968) -> (error out=w962:errorcluster)
            n669 = call <vilib>:"Clear Errors.vi"("error in (no error)"=w962) -> ()  [unwired: 5 in, 2 out]
          }
          frame #1 {
            n670 = global write "Variable glob generale.vi" "Acqui tout"(FALSE ("Acqui tout")) -> ()
            n671 = Request Deallocation(TRUE ("flag")) -> ()
          }
        }
      }
    }
    n672 = Wait (ms)(milliseconds to wait=u32 10 ("n millisecondes")) -> ()  [unwired: 1 out]
  }
